vi "NetScanner.vi"() -> ()   [LabVIEW 2026]
uses:
  <vilib>/Utility/file.llb/Read From Spreadsheet File (string).vi
  <vilib>/Platform/browser.llb/Open URL in Default Browser (path).vi
panel:
  in  "Open save folder":bool
  out "Load feedback":string
  in  "Load past data:":path
  out "Dummy \nsave:":bool
  in  "selectgraph2":u16(ring)=1 caption="Plot:" items=["p/p0", "Mach"]
  in  "Mach_Chan_Select":i16=1 caption="Calculate isentropic \nMach number\nfor channel:" min=1 max=15 step=1
  out "Chan_Mach":dbl caption="Isentropic Mach number:" format="%#_3g"
  out "Saved file:":string="p_1198.csv"
  out "Folder \nchange:":bool
  in  "Ones":T1={"Ch1"=TRUE, "Ch2"=TRUE, "Ch3"=TRUE, "Ch4"=TRUE, "Ch5"=TRUE, "Ch6"=TRUE, "Ch7"=TRUE, "Ch8"=TRUE, "Ch9"=TRUE, "Ch10"=TRUE, "Ch11"=TRUE, "Ch12"=TRUE, "Ch13"=TRUE, "Ch14"=TRUE, "Ch15"=TRUE, "Ch16"=TRUE} caption="Select Channel(s)"
  in  "Zeros":T1={"Ch1"=FALSE, "Ch2"=FALSE, "Ch3"=FALSE, "Ch4"=FALSE, "Ch5"=FALSE, "Ch6"=FALSE, "Ch7"=FALSE, "Ch8"=FALSE, "Ch9"=FALSE, "Ch10"=FALSE, "Ch11"=FALSE, "Ch12"=FALSE, "Ch13"=FALSE, "Ch14"=FALSE, "Ch15"=FALSE, "Ch16"=TRUE} caption="Select Channel(s)"
  in  "Toggle 1-15":bool=TRUE
  in  "unlock":bool
  in  "Runstop":bool
  out "File prefix:":string="p"
  out "Saved":bool
  in  "Folder path:":path=path "C:/Tim/March 2026/Cont pr"
  out "run time":timestamp=timestamp(3553599339.145414 s since 1904-01-01)
  in  "TCPref":refnum<k5>
  in  "Save":bool
  in  "channelselect":T1={"Ch1"=TRUE, "Ch2"=TRUE, "Ch3"=TRUE, "Ch4"=FALSE, "Ch5"=FALSE, "Ch6"=FALSE, "Ch7"=FALSE, "Ch8"=FALSE, "Ch9"=FALSE, "Ch10"=FALSE, "Ch11"=FALSE, "Ch12"=FALSE, "Ch13"=FALSE, "Ch14"=FALSE, "Ch15"=FALSE, "Ch16"=TRUE} caption="Select Channels:"
  out "datumtime":dbl=40.092
  out "datumpressure":dbl[](array[numeric])=[-0.0017857551574707031, 0.012584686279296875, -0.003287792205810547, -0.002514362335205078, 0.0002722740173339844, 9.584426879882812e-05, 0.0011773109436035156, -0.0024390220642089844, -0.0013475418090820312, 0.00286102294921875, 0.0024023056030273438, 0.0003457069396972656, -7.152557373046875e-06, -0.00193023681640625, 0.0019822120666503906, -0.00290679931640625]
  out "graphratio":cluster{"Y":dbl[], "Y":dbl[]}[](graph)
  out "graphpressure":cluster{"Y":dbl[], "Y":dbl[]}[](graph) caption="Pressure Traces"
  in  "unitselect":u16(ring)=3 caption="View Pressures as:" items=["Absolute [kPa]", "Absolute [psi]", "Gauge [kPa]", "Gauge [psi]"]
  out "datatimes":dbl[](array[numeric])=[0.063, 0.063, 0.063, 0.063, 0.064, 0.064, 0.072, 0.082, 0.092, 0.102, 0.112, 0.122, 0.132, 0.142, 0.152, 0.162, 0.172, 0.182, 0.192, 0.202, 0.212, 0.222, 0.232, 0.242, 0.252, 0.262, 0.272, 0.282, 0.292, 0.302, 0.313, 0.322, 0.333, 0.343, 0.353, 0.363, 0.373, 0.383, 0.393, 0.403, 0.413, 0.423, 0.433, 0.443, 0.453, 0.463, 0.473, 0.483, 0.493, 0.503, 0.513, 0.523, 0.533, 0.543, 0.553, 0.563, 0.573, 0.583, 0.593, 0.603, 0.613, 0.623, 0.633, 0.643, 0.653, 0.663, 0.673, 0.683, 0.693, 0.703, 0.713, 0.723, 0.734, 0.743, 0.754, 0.764, 0.774, 0.784, 0.794, 0.804, 0.814, 0.824, 0.834, 0.844, 0.854, 0.864, 0.874, 0.884, 0.894, 0.904, 0.914, 0.924, 0.934, 0.944, 0.954, 0.964, 0.974, 0.984, 0.994, 1.004, 1.014, 1.024, 1.034, 1.044, 1.054, 1.064, 1.074, 1.084, 1.094, 1.104, 1.114, 1.125, 1.134, 1.144, 1.154, 1.164, 1.194, 1.194, 1.195, 1.205, 1.215, 1.225, 1.235, 1.245, 1.255, 1.265, 1.275, 1.285, 1.295, 1.305, 1.315, 1.325, 1.335, 1.345, 1.355, 1.365, 1.375, 1.385, 1.395, 1.405, 1.415, 1.425, 1.435, 1.445, 1.455, 1.465, 1.476, 1.485, 1.495, 1.505, 1.516, 1.525, 1.535, 1.545, 1.556, 1.566, 1.576, 1.586, 1.596, 1.606, 1.616, 1.626, 1.636, 1.646, 1.656, 1.666, 1.676, 1.686, 1.696, 1.706, 1.716, 1.726, 1.736, 1.746, 1.756, 1.766, 1.776, 1.787, 1.797, 1.807, 1.817, 1.827, 1.837, 1.847, 1.857, 1.867, 1.877, 1.887, 1.897, 1.907, 1.917, 1.927, 1.937, 1.948, 1.958, 1.967, 1.978, 1.987, 1.998, 2.008, 2.018, 2.028, 2.038, 2.048, 2.058, 2.068, 2.078, 2.088, 2.098, 2.108, 2.118, 2.128, 2.138, 2.148, 2.158, 2.168, 2.178, 2.188, 2.198, 2.208, 2.218, 2.228, 2.238, 2.248, 2.258, 2.268, 2.278, 2.288, 2.298, 2.308, 2.318, 2.328, 2.338, 2.348, 2.359, 2.368, 2.379, 2.389, 2.398, 2.409, 2.419, 2.429, 2.439, 2.449, 2.459, 2.469, 2.479, 2.489, 2.499, 2.509, 2.519, 2.529, 2.539, 2.549, 2.559, 2.569, 2.579, 2.589, 2.599, 2.609, 2.619, 2.629, 2.639, 2.649, 2.659, 2.669, 2.679, 2.689, 2.699, 2.709, 2.719, 2.729, 2.739, 2.749, 2.759, 2.769, 2.78, 2.789, 2.8, 2.809, 2.82, 2.83, 2.84, 2.85, 2.86, 2.87, 2.88, 2.89, 2.9, 2.91, 2.92, 2.93, 2.94, 2.95, 2.96, 2.97, 2.98, 2.99, 3.0, 3.01, 3.02, 3.03, 3.04, 3.05, 3.06, 3.07, 3.08, 3.09, 3.1, 3.11, 3.12, 3.13, 3.14, 3.15, 3.16, 3.17, 3.181, 3.191, 3.2, 3.21, 3.22, 3.231, 3.241, 3.251, 3.261, 3.271, 3.281, 3.291, 3.301, 3.311, 3.321, 3.331, 3.341, 3.351, 3.361, 3.371, 3.381, 3.391, 3.401, 3.411, 3.421, 3.431, 3.441, 3.451, 3.461, 3.471, 3.481, 3.491, 3.501, 3.511, 3.521, 3.531, 3.541, 3.551, 3.561, 3.571, 3.582, 3.591, 3.601, 3.611, 3.621, 3.632, 3.642, 3.652, 3.662, 3.672, 3.682, 3.692, 3.702, 3.712, 3.722, 3.732, 3.742, 3.752, 3.762, 3.772, 3.782, 3.792, 3.802, 3.812, 3.822, 3.832, 3.842, 3.852, 3.862, 3.872, 3.882, 3.892, 3.902, 3.912, 3.922, 3.932, 3.942, 3.952, 3.962, 3.972, 3.982, 3.992, 4.003, 4.012, 4.022, 4.033, 4.043, 4.053, 4.063, 4.073, 4.083, 4.093, 4.103, 4.113, 4.123, 4.133, 4.143, 4.153, 4.163, 4.173, 4.183, 4.193, 4.203, 4.213, 4.223, 4.233, 4.243, 4.253, 4.263, 4.273, 4.283, 4.293, 4.303, 4.313, 4.323, 4.333, 4.343, 4.353, 4.363, 4.373, 4.383, 4.393, 4.403, 4.414, 4.423, 4.434, 4.443, 4.453, 4.464, 4.474, 4.484, 4.494, 4.504, 4.514, 4.524, 4.534, 4.544, 4.554, 4.564, 4.574, 4.584, 4.594, 4.604, 4.614, 4.624, 4.634, 4.644, 4.654, 4.664, 4.674, 4.684, 4.694, 4.704, 4.714, 4.724, 4.734, 4.744, 4.754, 4.764, 4.774, 4.785, 4.794, 4.804, 4.814, 4.824, 4.834, 4.844, 4.854, 4.864, 4.874, 4.885, 4.895, 4.905, 4.915, 4.925, 4.935, 4.945, 4.955, 4.965, 4.975, 4.985, 4.995, 5.005, 5.015, 5.025, 5.035, 5.045, 5.055, 5.065, 5.075, 5.085, 5.095, 5.105, 5.115, 5.125, 5.135, 5.145, 5.155, 5.165, 5.175, 5.185, 5.195, 5.205, 5.215, 5.225, 5.235, 5.245, 5.256, 5.265, 5.275, 5.286, 5.295, 5.306, 5.316, 5.326, 5.336, 5.346, 5.356, 5.366, 5.376, 5.386, 5.396, 5.406, 5.416, 5.426, 5.436, 5.446, 5.456, 5.466, 5.476, 5.486, 5.496, 5.506, 5.516, 5.526, 5.536, 5.546, 5.556, 5.566, 5.576, 5.586, 5.596, 5.606, 5.616, 5.626, 5.636, 5.646, 5.656, 5.666, 5.676, 5.687, 5.696, 5.707, 5.717, 5.727, 5.737, 5.747, 5.757, 5.767, 5.777, 5.787, 5.797, 5.807, 5.817, 5.827, 5.837, 5.847, 5.857, 5.867, 5.877, 5.887, 5.897, 5.907, 5.917, 5.927, 5.937, 5.947, 5.957, 5.967, 5.977, 5.987, 5.997, 6.007, 6.017, 6.027, 6.037, 6.047, 6.057, 6.068, 6.077, 6.088, 6.097, 6.108, 6.117, 6.128, 6.138, 6.148, 6.158, 6.168, 6.178, 6.188, 6.198, 6.208, 6.218, 6.228, 6.238, 6.248, 6.258, 6.268, 6.278, 6.288, 6.298, 6.308, 6.318, 6.328, 6.338, 6.348, 6.358, 6.368, 6.378, 6.388, 6.398, 6.408, 6.418, 6.428, 6.438, 6.448, 6.458, 6.468, 6.478, 6.489, 6.498, 6.508, 6.518, 6.529, 6.538, 6.549, 6.559, 6.569, 6.579, 6.589, 6.599, 6.609, 6.619, 6.629, 6.639, 6.649, 6.659, 6.669, 6.679, 6.689, 6.699, 6.709, 6.719, 6.729, 6.739, 6.749, 6.759, 6.769, 6.779, 6.789, 6.799, 6.809, 6.819, 6.829, 6.839, 6.849, 6.859, 6.869, 6.879, 6.89, 6.899, 6.909, 6.919, 6.93, 6.939, 6.95, 6.96, 6.97, 6.98, 6.99, 7.0, 7.01, 7.02, 7.03, 7.04, 7.05, 7.06, 7.07, 7.08, 7.09, 7.1, 7.11, 7.12, 7.13, 7.14, 7.15, 7.16, 7.17, 7.18, 7.19, 7.2, 7.21, 7.22, 7.23, 7.24, 7.25, 7.26, 7.27, 7.28, 7.29, 7.3, 7.31, 7.32, 7.331, 7.341, 7.351, 7.36, 7.37, 7.381, 7.391, 7.401, 7.411, 7.421, 7.431, 7.441, 7.451, 7.461, 7.471, 7.481, 7.491, 7.501, 7.511, 7.521, 7.531, 7.541, 7.551, 7.561, 7.571, 7.581, 7.591, 7.601, 7.611, 7.621, 7.631, 7.641, 7.651, 7.661, 7.671, 7.681, 7.691, 7.701, 7.711, 7.721, 7.731, 7.741, 7.751, 7.761, 7.772, 7.782, 7.792, 7.802, 7.812, 7.822, 7.832, 7.842, 7.852, 7.862, 7.872, 7.882, 7.892, 7.902, 7.912, 7.922, 7.932, 7.942, 7.952, 7.962, 7.972, 7.982, 7.992, 8.002, 8.012, 8.022, 8.032, 8.042, 8.052, 8.062, 8.072, 8.082, 8.092, 8.102, 8.112, 8.122, 8.132, 8.142, 8.152, 8.162, 8.173, 8.183, 8.193, 8.203, 8.213, 8.223, 8.233, 8.243, 8.253, 8.263, 8.273, 8.283, 8.293, 8.303, 8.313, 8.323, 8.333, 8.343, 8.353, 8.363, 8.373, 8.383, 8.393, 8.403, 8.413, 8.423, 8.433, 8.443, 8.453, 8.463, 8.473, 8.483, 8.493, 8.503, 8.513, 8.523, 8.533, 8.543, 8.553, 8.563, 8.573, 8.583, 8.594, 8.604, 8.614, 8.624, 8.634, 8.644, 8.654, 8.664, 8.674, 8.684, 8.694, 8.704, 8.714, 8.724, 8.734, 8.744, 8.754, 8.764, 8.774, 8.784, 8.794, 8.804, 8.814, 8.824, 8.834, 8.844, 8.854, 8.864, 8.874, 8.884, 8.894, 8.904, 8.914, 8.924, 8.934, 8.944, 8.954, 8.964, 8.974, 8.984, 8.995, 9.005, 9.015, 9.025, 9.035, 9.045, 9.055, 9.065, 9.075, 9.085, 9.095, 9.105, 9.115, 9.125, 9.135, 9.145, 9.155, 9.165, 9.175, 9.185, 9.195, 9.205, 9.215, 9.225, 9.235, 9.245, 9.255, 9.265, 9.275, 9.285, 9.295, 9.305, 9.315, 9.325, 9.335, 9.345, 9.355, 9.365, 9.375, 9.385, 9.396, 9.405, 9.416, 9.426, 9.436, 9.446, 9.456, 9.466, 9.476, 9.486, 9.496, 9.506, 9.516, 9.526, 9.536, 9.546, 9.556, 9.566, 9.576, 9.586, 9.596, 9.606, 9.616, 9.626, 9.636, 9.646, 9.656, 9.666, 9.676, 9.686, 9.696, 9.706, 9.716, 9.726, 9.736, 9.746, 9.756, 9.766, 9.776, 9.786, 9.797, 9.807, 9.816, 9.827, 9.837, 9.847, 9.857, 9.867, 9.877, 9.887, 9.897, 9.907, 9.917, 9.927, 9.937, 9.947, 9.957, 9.967, 9.977, 9.987, 9.997, 10.007, 10.017, 10.027, 10.037, 10.047, 10.057, 10.067, 10.077, 10.087, 10.097, 10.107, 10.117, 10.127, 10.137, 10.147, 10.157, 10.167, 10.177, 10.187, 10.198, 10.207, 10.217, 10.227, 10.237, 10.248, 10.258, 10.268, 10.278, 10.288, 10.298, 10.308, 10.318, 10.328, 10.338, 10.348, 10.358, 10.368, 10.378, 10.388, 10.398, 10.408, 10.418, 10.428, 10.438, 10.448, 10.458, 10.468, 10.478, 10.488, 10.498, 10.508, 10.518, 10.528, 10.538, 10.548, 10.558, 10.568, 10.578, 10.588, 10.599, 10.608, 10.618, 10.628, 10.638, 10.649, 10.659, 10.669, 10.679, 10.689, 10.699, 10.709, 10.719, 10.729, 10.739, 10.749, 10.759, 10.769, 10.779, 10.789, 10.799, 10.809, 10.819, 10.829, 10.839, 10.849, 10.859, 10.869, 10.879, 10.889, 10.899, 10.909, 10.919, 10.929, 10.939, 10.949, 10.959, 10.969, 10.979, 10.989, 11.0, 11.009, 11.019, 11.029, 11.039, 11.05, 11.06, 11.07, 11.08, 11.09, 11.1, 11.11, 11.12, 11.13, 11.14, 11.15, 11.16, 11.17, 11.18, 11.19, 11.2, 11.21, 11.22, 11.23, 11.24, 11.25, 11.26, 11.27, 11.28, 11.29, 11.3, 11.31, 11.32, 11.33, 11.34, 11.35, 11.36, 11.37, 11.38, 11.39, 11.4, 11.41, 11.42, 11.43, 11.44, 11.45, 11.46, 11.47, 11.481, 11.491, 11.501, 11.511, 11.521, 11.531, 11.541, 11.551, 11.561, 11.571, 11.581, 11.591, 11.601, 11.611, 11.621, 11.631, 11.641, 11.651, 11.661, 11.671, 11.681, 11.691, 11.701, 11.711, 11.721, 11.731, 11.741, 11.751, 11.761, 11.771, 11.781, 11.791, 11.801, 11.811, 11.821, 11.831, 11.841, 11.851, 11.861, 11.871, 11.882, 11.892, 11.902, 11.912, 11.922, 11.932, 11.942, 11.952, 11.962, 11.972, 11.982, 11.992, 12.002, 12.012, 12.022, 12.032, 12.042, 12.052, 12.062, 12.072, 12.082, 12.092, 12.102, 12.112, 12.122, 12.132, 12.142, 12.152, 12.162, 12.172, 12.182, 12.192, 12.202, 12.212, 12.222, 12.232, 12.243, 12.252, 12.262, 12.272, 12.282, 12.292, 12.303, 12.313, 12.323, 12.333, 12.343, 12.353, 12.363, 12.373, 12.383, 12.393, 12.403, 12.413, 12.423, 12.433, 12.443, 12.453, 12.463, 12.473, 12.483, 12.493, 12.503, 12.513, 12.523, 12.533, 12.543, 12.553, 12.563, 12.573, 12.583, 12.593, 12.603, 12.613, 12.623, 12.633, 12.643, 12.653, 12.663, 12.673, 12.684, 12.694, 12.704, 12.714, 12.724, 12.734, 12.744, 12.754, 12.764, 12.774, 12.784, 12.794, 12.804, 12.814, 12.824, 12.834, 12.844, 12.854, 12.864, 12.874, 12.884, 12.894, 12.904, 12.914, 12.924, 12.934, 12.944, 12.954, 12.964, 12.974, 12.984, 12.994, 13.004, 13.014, 13.024, 13.034, 13.044, 13.054, 13.064, 13.074, 13.084, 13.094, 13.104, 13.115, 13.125, 13.135, 13.145, 13.155, 13.165, 13.175, 13.185, 13.195, 13.205, 13.215, 13.225, 13.235, 13.245, 13.255, 13.265, 13.275, 13.285, 13.295, 13.305, 13.315, 13.325, 13.335, 13.345, 13.355, 13.365, 13.375, 13.385, 13.395, 13.405, 13.415, 13.425, 13.435, 13.445, 13.455, 13.465, 13.475, 13.485, 13.495, 13.506, 13.515, 13.525, 13.536, 13.546, 13.556, 13.566, 13.576, 13.586, 13.596, 13.606, 13.616, 13.626, 13.636, 13.646, 13.656, 13.666, 13.676, 13.686, 13.696, 13.706, 13.716, 13.726, 13.736, 13.746, 13.756, 13.766, 13.776, 13.786, 13.796, 13.806, 13.816, 13.826, 13.836, 13.846, 13.856, 13.866, 13.876, 13.886, 13.896, 13.906, 13.916, 13.926, 13.936, 13.946, 13.956, 13.966, 13.977, 13.987, 13.997, 14.007, 14.017, 14.027, 14.037, 14.047, 14.057, 14.067, 14.077, 14.087, 14.097, 14.107, 14.117, 14.127, 14.137, 14.147, 14.157, 14.167, 14.177, 14.187, 14.197, 14.207, 14.217, 14.227, 14.237, 14.247, 14.257, 14.267, 14.277, 14.287, 14.297, 14.307, 14.317, 14.327, 14.338, 14.348, 14.357, 14.368, 14.378, 14.388, 14.398, 14.408, 14.418, 14.428, 14.438, 14.448, 14.458, 14.468, 14.478, 14.488, 14.498, 14.508, 14.518, 14.528, 14.538, 14.548, 14.558, 14.568, 14.578, 14.588, 14.598, 14.608, 14.618, 14.628, 14.638, 14.648, 14.658, 14.668, 14.678, 14.688, 14.698, 14.708, 14.718, 14.728, 14.739, 14.749, 14.759, 14.769, 14.779, 14.789, 14.799, 14.809, 14.819, 14.829, 14.839, 14.849, 14.859, 14.869, 14.879, 14.889, 14.899, 14.909, 14.919, 14.929, 14.939, 14.949, 14.959, 14.969, 14.979, 14.989, 14.999, 15.009, 15.019, 15.029, 15.039, 15.049, 15.059, 15.069, 15.079, 15.089, 15.099, 15.109, 15.12, 15.13, 15.14, 15.15, 15.16, 15.17, 15.18, 15.19, 15.2, 15.21, 15.22, 15.23, 15.24, 15.25, 15.26, 15.27, 15.28, 15.29, 15.3, 15.31, 15.32, 15.33, 15.34, 15.35, 15.36, 15.37, 15.38, 15.39, 15.4, 15.446, 15.446, 15.446, 15.446, 15.45, 15.46, 15.47, 15.48, 15.49, 15.5, 15.51, 15.52, 15.53, 15.54, 15.55, 15.56, 15.571, 15.581, 15.591, 15.601, 15.611, 15.621, 15.631, 15.641, 15.651, 15.661, 15.671, 15.681, 15.691, 15.701, 15.711, 15.721, 15.731, 15.741, 15.751, 15.761, 15.771, 15.781, 15.791, 15.801, 15.811, 15.821, 15.831, 15.841, 15.851, 15.861, 15.871, 15.881, 15.891, 15.901, 15.911, 15.922, 15.931, 15.941, 15.951, 15.962, 15.972, 15.982, 15.992, 16.002, 16.012, 16.022, 16.032, 16.042, 16.052, 16.062, 16.072, 16.082, 16.092, 16.102, 16.112, 16.122, 16.132, 16.142, 16.152, 16.162, 16.172, 16.182, 16.192, 16.202, 16.212, 16.222, 16.232, 16.242, 16.252, 16.262, 16.272, 16.282, 16.292, 16.302, 16.312, 16.322, 16.332, 16.342, 16.352, 16.362, 16.372, 16.382, 16.392, 16.402, 16.413, 16.423, 16.433, 16.443, 16.453, 16.463, 16.473, 16.483, 16.493, 16.503, 16.513, 16.523, 16.533, 16.543, 16.553, 16.563, 16.573, 16.583, 16.593, 16.603, 16.613, 16.623, 16.633, 16.643, 16.653, 16.663, 16.673, 16.683, 16.693, 16.703, 16.713, 16.723, 16.733, 16.743, 16.753, 16.763, 16.773, 16.784, 16.793, 16.804, 16.814, 16.824, 16.834, 16.844, 16.854, 16.864, 16.874, 16.884, 16.894, 16.904, 16.914, 16.924, 16.934, 16.944, 16.954, 16.964, 16.974, 16.984, 16.994, 17.004, 17.014, 17.024, 17.034, 17.044, 17.054, 17.064, 17.074, 17.084, 17.094, 17.104, 17.114, 17.124, 17.134, 17.144, 17.154, 17.164, 17.174, 17.184, 17.194, 17.205, 17.215, 17.225, 17.235, 17.245, 17.255, 17.264, 17.275, 17.285, 17.295, 17.305, 17.315, 17.325, 17.335, 17.345, 17.355, 17.365, 17.375, 17.385, 17.395, 17.405, 17.415, 17.425, 17.435, 17.445, 17.455, 17.465, 17.475, 17.485, 17.495, 17.505, 17.515, 17.525, 17.535, 17.545, 17.556, 17.565, 17.575, 17.586, 17.596, 17.605, 17.616, 17.626, 17.636, 17.646, 17.656, 17.666, 17.676, 17.686, 17.696, 17.706, 17.716, 17.726, 17.736, 17.746, 17.756, 17.766, 17.776, 17.786, 17.796, 17.806, 17.816, 17.826, 17.836, 17.846, 17.856, 17.866, 17.876, 17.886, 17.896, 17.906, 17.916, 17.926, 17.936, 17.946, 17.957, 17.966, 17.976, 17.986, 17.996, 18.007, 18.017, 18.027, 18.037, 18.047, 18.057, 18.067, 18.077, 18.087, 18.097, 18.107, 18.117, 18.127, 18.137, 18.147, 18.157, 18.167, 18.177, 18.187, 18.197, 18.207, 18.217, 18.227, 18.237, 18.247, 18.257, 18.267, 18.277, 18.287, 18.297, 18.307, 18.317, 18.327, 18.337, 18.347, 18.357, 18.367, 18.377, 18.387, 18.397, 18.407, 18.418, 18.427, 18.438, 18.447, 18.457, 18.467, 18.478, 18.488, 18.498, 18.508, 18.518, 18.528, 18.538, 18.548, 18.558, 18.568, 18.578, 18.588, 18.598, 18.608, 18.618, 18.628, 18.638, 18.648, 18.658, 18.668, 18.678, 18.688, 18.698, 18.708, 18.718, 18.728, 18.738, 18.748, 18.758, 18.768, 18.778, 18.788, 18.798, 18.808, 18.818, 18.828, 18.838, 18.848, 18.858, 18.868, 18.878, 18.889, 18.899, 18.909, 18.919, 18.929, 18.939, 18.949, 18.959, 18.969, 18.979, 18.989, 18.999, 19.009, 19.019, 19.029, 19.039, 19.049, 19.059, 19.069, 19.079, 19.089, 19.099, 19.109, 19.119, 19.129, 19.139, 19.149, 19.159, 19.169, 19.179, 19.189, 19.199, 19.209, 19.219, 19.23, 19.24, 19.249, 19.259, 19.27, 19.28, 19.29, 19.301, 19.31, 19.321, 19.331, 19.341, 19.351, 19.361, 19.371, 19.381, 19.391, 19.401, 19.411, 19.421, 19.431, 19.441, 19.451, 19.461, 19.471, 19.481, 19.491, 19.501, 19.511, 19.521, 19.531, 19.541, 19.551, 19.561, 19.571, 19.581, 19.591, 19.601, 19.611, 19.622, 19.631, 19.641, 19.651, 19.661, 19.671, 19.681, 19.691, 19.701, 19.711, 19.722, 19.731, 19.741, 19.751, 19.762, 19.772, 19.782, 19.792, 19.802, 19.812, 19.822, 19.832, 19.842, 19.852, 19.862, 19.872, 19.882, 19.892, 19.902, 19.912, 19.922, 19.932, 19.942, 19.952, 19.962, 19.972, 19.982, 19.992, 20.002, 20.012, 20.022, 20.032, 20.042, 20.052, 20.062, 20.072, 20.082, 20.092, 20.102, 20.112, 20.122, 20.132, 20.143, 20.153, 20.163, 20.173, 20.183, 20.193, 20.203, 20.213, 20.223, 20.233, 20.243, 20.253, 20.263, 20.273, 20.283, 20.293, 20.303, 20.313, 20.323, 20.333, 20.343, 20.353, 20.363, 20.373, 20.383, 20.393, 20.403, 20.413, 20.423, 20.433, 20.443, 20.453, 20.463, 20.473, 20.483, 20.493, 20.503, 20.513, 20.523, 20.533, 20.544, 20.554, 20.564, 20.574, 20.584, 20.594, 20.604, 20.614, 20.624, 20.634, 20.644, 20.654, 20.664, 20.674, 20.684, 20.694, 20.704, 20.714, 20.724, 20.734, 20.744, 20.754, 20.764, 20.774, 20.784, 20.794, 20.804, 20.814, 20.824, 20.834, 20.844, 20.854, 20.864, 20.874, 20.884, 20.894, 20.904, 20.914, 20.925, 20.934, 20.944, 20.954, 20.964, 20.975, 20.985, 20.995, 21.005, 21.015, 21.025, 21.035, 21.045, 21.055, 21.065, 21.075, 21.085, 21.095, 21.105, 21.115, 21.125, 21.135, 21.145, 21.155, 21.165, 21.175, 21.185, 21.195, 21.205, 21.215, 21.225, 21.235, 21.245, 21.255, 21.265, 21.275, 21.285, 21.295, 21.305, 21.315, 21.325, 21.335, 21.345, 21.355, 21.366, 21.376, 21.386, 21.396, 21.406, 21.416, 21.426, 21.436, 21.446, 21.456, 21.466, 21.476, 21.486, 21.496, 21.506, 21.516, 21.526, 21.536, 21.546, 21.556, 21.566, 21.576, 21.586, 21.596, 21.606, 21.616, 21.626, 21.636, 21.646, 21.656, 21.666, 21.676, 21.686, 21.696, 21.706, 21.716, 21.726, 21.736, 21.746, 21.756, 21.766, 21.776, 21.786, 21.796, 21.806, 21.817, 21.826, 21.837, 21.847, 21.857, 21.867, 21.877, 21.887, 21.897, 21.907, 21.917, 21.927, 21.937, 21.947, 21.957, 21.967, 21.977, 21.987, 21.997, 22.007, 22.017, 22.027, 22.037, 22.047, 22.057, 22.067, 22.077, 22.087, 22.097, 22.107, 22.118, 22.127, 22.137, 22.147, 22.157, 22.167, 22.177, 22.188, 22.198, 22.208, 22.218, 22.228, 22.238, 22.248, 22.258, 22.268, 22.278, 22.288, 22.298, 22.308, 22.318, 22.328, 22.338, 22.348, 22.358, 22.368, 22.378, 22.388, 22.398, 22.408, 22.418, 22.428, 22.438, 22.448, 22.458, 22.468, 22.478, 22.488, 22.498, 22.508, 22.518, 22.528, 22.538, 22.548, 22.558, 22.568, 22.579, 22.589, 22.599, 22.609, 22.619, 22.629, 22.639, 22.649, 22.659, 22.669, 22.679, 22.689, 22.699, 22.709, 22.719, 22.729, 22.739, 22.749, 22.759, 22.769, 22.779, 22.789, 22.799, 22.809, 22.819, 22.829, 22.839, 22.849, 22.859, 22.869, 22.879, 22.889, 22.899, 22.909, 22.919, 22.929, 22.939, 22.949, 22.959, 22.969, 22.979, 22.989, 22.999, 23.009, 23.019, 23.03, 23.039, 23.049, 23.059, 23.07, 23.08, 23.09, 23.1, 23.11, 23.12, 23.13, 23.14, 23.15, 23.16, 23.17, 23.18, 23.19, 23.2, 23.21, 23.22, 23.23, 23.24, 23.25, 23.26, 23.27, 23.28, 23.29, 23.3, 23.31, 23.32, 23.33, 23.34, 23.35, 23.36, 23.37, 23.38, 23.39, 23.4, 23.41, 23.42, 23.43, 23.441, 23.45, 23.461, 23.471, 23.481, 23.491, 23.501, 23.511, 23.521, 23.531, 23.541, 23.551, 23.561, 23.571, 23.581, 23.591, 23.601, 23.611, 23.621, 23.631, 23.641, 23.651, 23.661, 23.671, 23.681, 23.691, 23.701, 23.711, 23.721, 23.731, 23.741, 23.751, 23.761, 23.771, 23.781, 23.791, 23.801, 23.811, 23.821, 23.831, 23.841, 23.851, 23.861, 23.871, 23.882, 23.892, 23.902, 23.912, 23.922, 23.932, 23.942, 23.952, 23.962, 23.972, 23.982, 23.992, 24.002, 24.012, 24.022, 24.032, 24.042, 24.052, 24.062, 24.072, 24.082, 24.092, 24.102, 24.112, 24.122, 24.132, 24.142, 24.152, 24.162, 24.172, 24.182, 24.192, 24.202, 24.212, 24.222, 24.232, 24.242, 24.252, 24.262, 24.272, 24.282, 24.292, 24.303, 24.313, 24.323, 24.333, 24.343, 24.353, 24.363, 24.373, 24.383, 24.393, 24.403, 24.413, 24.423, 24.433, 24.443, 24.453, 24.463, 24.473, 24.483, 24.493, 24.503, 24.513, 24.523, 24.533, 24.543, 24.553, 24.563, 24.573, 24.583, 24.593, 24.603, 24.613, 24.623, 24.633, 24.643, 24.654, 24.663, 24.674, 24.684, 24.693, 24.703, 24.714, 24.724, 24.734, 24.744, 24.754, 24.764, 24.774, 24.784, 24.794, 24.804, 24.814, 24.824, 24.834, 24.844, 24.854, 24.864, 24.874, 24.884, 24.894, 24.904, 24.914, 24.924, 24.934, 24.944, 24.954, 24.964, 24.974, 24.984, 24.994, 25.004, 25.014, 25.024, 25.034, 25.044, 25.054, 25.064, 25.075, 25.084, 25.094, 25.105, 25.115, 25.125, 25.135, 25.145, 25.155, 25.165, 25.175, 25.185, 25.195, 25.205, 25.215, 25.225, 25.235, 25.245, 25.255, 25.265, 25.275, 25.285, 25.295, 25.305, 25.315, 25.325, 25.335, 25.345, 25.355, 25.365, 25.375, 25.385, 25.395, 25.405, 25.415, 25.425, 25.435, 25.445, 25.456, 25.466, 25.476, 25.486, 25.496, 25.506, 25.516, 25.526, 25.536, 25.546, 25.556, 25.566, 25.576, 25.586, 25.596, 25.606, 25.616, 25.626, 25.636, 25.646, 25.656, 25.666, 25.676, 25.686, 25.696, 25.706, 25.716, 25.726, 25.736, 25.746, 25.756, 25.766, 25.776, 25.786, 25.796, 25.806, 25.816, 25.826, 25.836, 25.846, 25.856, 25.866, 25.876, 25.886, 25.896, 25.907, 25.916, 25.927, 25.937, 25.947, 25.957, 25.967, 25.977, 25.987, 25.997, 26.007, 26.017, 26.027, 26.037, 26.047, 26.057, 26.067, 26.077, 26.087, 26.097, 26.107, 26.117, 26.127, 26.137, 26.147, 26.157, 26.167, 26.177, 26.187, 26.197, 26.207, 26.217, 26.227, 26.237, 26.247, 26.257, 26.267, 26.277, 26.287, 26.297, 26.307, 26.317, 26.328, 26.338, 26.348, 26.358, 26.367, 26.378, 26.388, 26.398, 26.408, 26.418, 26.428, 26.438, 26.448, 26.458, 26.468, 26.478, 26.488, 26.498, 26.508, 26.518, 26.528, 26.538, 26.548, 26.558, 26.568, 26.578, 26.588, 26.598, 26.608, 26.618, 26.628, 26.638, 26.648, 26.658, 26.668, 26.678, 26.688, 26.698, 26.708, 26.718, 26.728, 26.738, 26.748, 26.758, 26.769, 26.779, 26.789, 26.799, 26.809, 26.819, 26.829, 26.839, 26.849, 26.859, 26.869, 26.879, 26.889, 26.899, 26.909, 26.919, 26.929, 26.939, 26.949, 26.959, 26.969, 26.979, 26.989, 26.999, 27.009, 27.019, 27.029, 27.039, 27.049, 27.059, 27.069, 27.079, 27.089, 27.099, 27.109, 27.119, 27.129, 27.139, 27.149, 27.159, 27.169, 27.18, 27.19, 27.2, 27.209, 27.22, 27.23, 27.24, 27.25, 27.26, 27.27, 27.28, 27.29, 27.3, 27.31, 27.321, 27.33, 27.34, 27.35, 27.36, 27.37, 27.38, 27.39, 27.4, 27.41, 27.42, 27.43, 27.44, 27.45, 27.46, 27.47, 27.48, 27.49, 27.5, 27.51, 27.52, 27.53, 27.54, 27.55, 27.56, 27.57, 27.58, 27.591, 27.601, 27.611, 27.62, 27.631, 27.641, 27.651, 27.661, 27.671, 27.681, 27.691, 27.701, 27.713, 27.721, 27.731, 27.741, 27.751, 27.761, 27.771, 27.781, 27.791, 27.801, 27.811, 27.821, 27.831, 27.841, 27.851, 27.861, 27.871, 27.881, 27.891, 27.901, 27.911, 27.921, 27.931, 27.941, 27.951, 27.961, 27.971, 27.981, 27.991, 28.002, 28.011, 28.021, 28.031, 28.042, 28.052, 28.062, 28.072, 28.082, 28.092, 28.102, 28.112, 28.122, 28.132, 28.142, 28.152, 28.162, 28.172, 28.182, 28.192, 28.202, 28.212, 28.222, 28.232, 28.242, 28.252, 28.262, 28.272, 28.282, 28.292, 28.302, 28.312, 28.322, 28.332, 28.342, 28.352, 28.362, 28.372, 28.382, 28.392, 28.402, 28.412, 28.423, 28.432, 28.443, 28.452, 28.463, 28.473, 28.483, 28.493, 28.503, 28.513, 28.523, 28.533, 28.543, 28.553, 28.563, 28.573, 28.583, 28.593, 28.603, 28.613, 28.623, 28.633, 28.643, 28.653, 28.663, 28.673, 28.683, 28.693, 28.703, 28.713, 28.723, 28.733, 28.743, 28.753, 28.763, 28.774, 28.783, 28.793, 28.803, 28.814, 28.824, 28.833, 28.843, 28.854, 28.864, 28.874, 28.884, 28.894, 28.904, 28.914, 28.924, 28.934, 28.944, 28.954, 28.964, 28.974, 28.984, 28.994, 29.004, 29.014, 29.024, 29.034, 29.044, 29.054, 29.064, 29.074, 29.084, 29.094, 29.104, 29.114, 29.124, 29.134, 29.144, 29.154, 29.165, 29.174, 29.185, 29.195, 29.205, 29.215, 29.225, 29.235, 29.245, 29.255, 29.265, 29.275, 29.285, 29.295, 29.305, 29.315, 29.325, 29.335, 29.345, 29.355, 29.365, 29.375, 29.385, 29.395, 29.405, 29.415, 29.425, 29.435, 29.445, 29.455, 29.465, 29.475, 29.485, 29.495, 29.505, 29.515, 29.525, 29.535, 29.545, 29.556, 29.565, 29.575, 29.586, 29.596, 29.606, 29.616, 29.626, 29.636, 29.646, 29.656, 29.666, 29.676, 29.686, 29.696, 29.706, 29.716, 29.726, 29.736, 29.746, 29.756, 29.766, 29.776, 29.786, 29.796, 29.806, 29.816, 29.826, 29.836, 29.846, 29.856, 29.866, 29.876, 29.886, 29.896, 29.906, 29.916, 29.926, 29.936, 29.946, 29.957, 29.966, 29.976, 29.986, 29.996, 30.006, 30.017, 30.027, 30.037, 30.047, 30.057, 30.067, 30.077, 30.087, 30.097, 30.107, 30.117, 30.127, 30.137, 30.147, 30.157, 30.167, 30.177, 30.187, 30.197, 30.207, 30.217, 30.227, 30.237, 30.247, 30.257, 30.267, 30.277, 30.287, 30.297, 30.308, 30.317, 30.327, 30.337, 30.347, 30.358, 30.367, 30.378, 30.388, 30.398, 30.408, 30.417, 30.428, 30.438, 30.448, 30.458, 30.468, 30.478, 30.488, 30.498, 30.508, 30.518, 30.528, 30.538, 30.548, 30.558, 30.568, 30.578, 30.588, 30.598, 30.608, 30.618, 30.628, 30.638, 30.648, 30.658, 30.668, 30.678, 30.688, 30.698, 30.708, 30.718, 30.728, 30.738, 30.748, 30.758, 30.768, 30.778, 30.788, 30.798, 30.808, 30.818, 30.829, 30.839, 30.849, 30.859, 30.869, 30.879, 30.889, 30.899, 30.909, 30.919, 30.929, 30.939, 30.949, 30.959, 30.969, 30.979, 30.989, 30.999, 31.009, 31.019, 31.029, 31.039, 31.049, 31.059, 31.069, 31.079, 31.089, 31.099, 31.109, 31.119, 31.129, 31.139, 31.149, 31.159, 31.169, 31.179, 31.189, 31.199, 31.21, 31.219, 31.23, 31.24, 31.25, 31.26, 31.269, 31.28, 31.29, 31.3, 31.31, 31.32, 31.33, 31.34, 31.35, 31.36, 31.37, 31.38, 31.39, 31.4, 31.41, 31.42, 31.43, 31.44, 31.45, 31.46, 31.47, 31.48, 31.49, 31.5, 31.51, 31.52, 31.53, 31.54, 31.55, 31.56, 31.57, 31.58, 31.59, 31.6, 31.61, 31.62, 31.63, 31.64, 31.651, 31.661, 31.671, 31.681, 31.691, 31.701, 31.711, 31.721, 31.731, 31.741, 31.751, 31.761, 31.771, 31.781, 31.791, 31.801, 31.811, 31.821, 31.831, 31.841, 31.851, 31.861, 31.871, 31.881, 31.891, 31.901, 31.911, 31.921, 31.932, 31.941, 31.951, 31.961, 31.971, 31.981, 31.991, 32.001, 32.011, 32.021, 32.031, 32.041, 32.051, 32.062, 32.072, 32.082, 32.092, 32.102, 32.112, 32.122, 32.132, 32.142, 32.152, 32.162, 32.172, 32.182, 32.192, 32.202, 32.212, 32.222, 32.232, 32.242, 32.252, 32.262, 32.272, 32.282, 32.292, 32.302, 32.312, 32.322, 32.332, 32.342, 32.352, 32.363, 32.372, 32.382, 32.392, 32.402, 32.412, 32.422, 32.432, 32.442, 32.452, 32.462, 32.472, 32.482, 32.492, 32.502, 32.512, 32.523, 32.533, 32.543, 32.553, 32.562, 32.573, 32.583, 32.593, 32.603, 32.613, 32.623, 32.633, 32.643, 32.653, 32.663, 32.673, 32.683, 32.693, 32.703, 32.713, 32.723, 32.733, 32.743, 32.753, 32.763, 32.773, 32.783, 32.793, 32.803, 32.813, 32.823, 32.833, 32.843, 32.853, 32.863, 32.873, 32.884, 32.894, 32.904, 32.914, 32.924, 32.934, 32.944, 32.954, 32.964, 32.974, 32.984, 32.994, 33.004, 33.014, 33.024, 33.034, 33.044, 33.054, 33.064, 33.074, 33.084, 33.094, 33.104, 33.114, 33.124, 33.134, 33.144, 33.154, 33.164, 33.174, 33.184, 33.194, 33.204, 33.214, 33.224, 33.234, 33.244, 33.254, 33.264, 33.274, 33.284, 33.294, 33.304, 33.315, 33.324, 33.334, 33.344, 33.355, 33.365, 33.375, 33.385, 33.395, 33.405, 33.415, 33.425, 33.435, 33.445, 33.455, 33.465, 33.475, 33.485, 33.495, 33.505, 33.515, 33.525, 33.535, 33.545, 33.555, 33.565, 33.575, 33.585, 33.595, 33.605, 33.615, 33.625, 33.635, 33.645, 33.655, 33.665, 33.675, 33.685, 33.695, 33.705, 33.715, 33.725, 33.735, 33.745, 33.756, 33.765, 33.775, 33.786, 33.796, 33.806, 33.816, 33.826, 33.836, 33.846, 33.856, 33.866, 33.876, 33.886, 33.896, 33.906, 33.916, 33.926, 33.936, 33.946, 33.956, 33.966, 33.976, 33.986, 33.996, 34.006, 34.016, 34.026, 34.036, 34.046, 34.056, 34.066, 34.076, 34.086, 34.096, 34.106, 34.116, 34.126, 34.136, 34.146, 34.156, 34.166, 34.176, 34.186, 34.197, 34.206, 34.216, 34.226, 34.237, 34.247, 34.257, 34.267, 34.277, 34.287, 34.297, 34.307, 34.317, 34.327, 34.337, 34.347, 34.357, 34.367, 34.377, 34.387, 34.397, 34.407, 34.417, 34.427, 34.437, 34.447, 34.457, 34.467, 34.477, 34.487, 34.497, 34.507, 34.517, 34.527, 34.537, 34.547, 34.557, 34.567, 34.577, 34.587, 34.597, 34.607, 34.617, 34.628, 34.638, 34.648, 34.658, 34.668, 34.678, 34.688, 34.698, 34.708, 34.718, 34.728, 34.738, 34.748, 34.758, 34.768, 34.778, 34.788, 34.798, 34.808, 34.818, 34.828, 34.838, 34.848, 34.858, 34.868, 34.878, 34.888, 34.898, 34.908, 34.918, 34.928, 34.938, 34.948, 34.958, 34.968, 34.978, 34.988, 34.998, 35.008, 35.018, 35.029, 35.039, 35.049, 35.059, 35.069, 35.079, 35.089, 35.099, 35.109, 35.119, 35.129, 35.139, 35.149, 35.159, 35.169, 35.179, 35.189, 35.199, 35.209, 35.219, 35.229, 35.239, 35.249, 35.259, 35.269, 35.279, 35.289, 35.299, 35.309, 35.319, 35.329, 35.339, 35.349, 35.359, 35.369, 35.379, 35.389, 35.399, 35.409, 35.419, 35.429, 35.44, 35.449, 35.46, 35.469, 35.48, 35.49, 35.5, 35.51, 35.52, 35.53, 35.54, 35.55, 35.56, 35.57, 35.58, 35.59, 35.6, 35.61, 35.62, 35.63, 35.64, 35.65, 35.66, 35.671, 35.68, 35.69, 35.7, 35.71, 35.72, 35.73, 35.74, 35.75, 35.761, 35.77, 35.781, 35.791, 35.801, 35.811, 35.821, 35.831, 35.841, 35.85, 35.861, 35.871, 35.881, 35.891, 35.901, 35.911, 35.921, 35.931, 35.941, 35.951, 35.961, 35.971, 35.981, 35.991, 36.001, 36.011, 36.021, 36.031, 36.041, 36.051, 36.061, 36.071, 36.081, 36.091, 36.101, 36.111, 36.121, 36.131, 36.141, 36.151, 36.161, 36.171, 36.181, 36.191, 36.201, 36.211, 36.222, 36.231, 36.241, 36.252, 36.262, 36.272, 36.282, 36.292, 36.302, 36.312, 36.322, 36.332, 36.342, 36.352, 36.362, 36.372, 36.382, 36.392, 36.402, 36.412, 36.422, 36.432, 36.442, 36.452, 36.462, 36.472, 36.482, 36.492, 36.502, 36.512, 36.522, 36.532, 36.542, 36.552, 36.562, 36.572, 36.582, 36.592, 36.602, 36.612, 36.622, 36.632, 36.642, 36.653, 36.663, 36.673, 36.682, 36.693, 36.703, 36.713, 36.723, 36.733, 36.743, 36.754, 36.764, 36.774, 36.784, 36.794, 36.804, 36.814, 36.824, 36.834, 36.844, 36.854, 36.864, 36.874, 36.884, 36.894, 36.904, 36.914, 36.924, 36.934, 36.944, 36.954, 36.964, 36.974, 36.984, 36.994, 37.004, 37.014, 37.024, 37.034, 37.044, 37.054, 37.064, 37.074, 37.084, 37.095, 37.105, 37.115, 37.125, 37.135, 37.145, 37.155, 37.165, 37.175, 37.185, 37.195, 37.205, 37.215, 37.225, 37.235, 37.245, 37.255, 37.265, 37.275, 37.285, 37.295, 37.305, 37.315, 37.325, 37.335, 37.345, 37.355, 37.365, 37.375, 37.385, 37.395, 37.405, 37.415, 37.425, 37.435, 37.446, 37.455, 37.465, 37.476, 37.486, 37.496, 37.506, 37.516, 37.526, 37.536, 37.546, 37.556, 37.566, 37.576, 37.586, 37.596, 37.606, 37.616, 37.626, 37.636, 37.646, 37.656, 37.666, 37.676, 37.686, 37.696, 37.706, 37.716, 37.726, 37.736, 37.746, 37.756, 37.766, 37.776, 37.786, 37.796, 37.806, 37.816, 37.826, 37.836, 37.846, 37.856, 37.866, 37.877, 37.886, 37.897, 37.907, 37.917, 37.927, 37.937, 37.947, 37.957, 37.967, 37.977, 37.987, 37.997, 38.007, 38.017, 38.027, 38.037, 38.047, 38.057, 38.067, 38.077, 38.087, 38.097, 38.107, 38.117, 38.127, 38.137, 38.147, 38.157, 38.167, 38.177, 38.187, 38.197, 38.207, 38.217, 38.227, 38.237, 38.247, 38.257, 38.267, 38.277, 38.287, 38.297, 38.307, 38.318, 38.328, 38.338, 38.348, 38.358, 38.368, 38.378, 38.388, 38.398, 38.408, 38.418, 38.428, 38.438, 38.448, 38.458, 38.468, 38.478, 38.488, 38.498, 38.508, 38.518, 38.528, 38.538, 38.548, 38.558, 38.568, 38.578, 38.588, 38.598, 38.608, 38.618, 38.628, 38.638, 38.648, 38.658, 38.668, 38.678, 38.688, 38.698, 38.708, 38.719, 38.729, 38.739, 38.749, 38.759, 38.769, 38.779, 38.789, 38.799, 38.809, 38.819, 38.829, 38.839, 38.849, 38.859, 38.869, 38.879, 38.889, 38.899, 38.909, 38.919, 38.929, 38.939, 38.949, 38.959, 38.969, 38.979, 38.989, 38.999, 39.009, 39.019, 39.029, 39.039, 39.049, 39.059, 39.069, 39.079, 39.089, 39.099, 39.109, 39.119, 39.129, 39.14, 39.15, 39.16, 39.17, 39.18, 39.19, 39.2, 39.21, 39.22, 39.23, 39.24, 39.25, 39.26, 39.27, 39.28, 39.29, 39.3, 39.31, 39.32, 39.33, 39.34, 39.35, 39.36, 39.37, 39.38, 39.39, 39.4, 39.41, 39.42, 39.43, 39.44, 39.45, 39.46, 39.47, 39.48, 39.49, 39.501, 39.51, 39.52, 39.53, 39.541, 39.551, 39.561, 39.571, 39.581, 39.591, 39.601, 39.611, 39.621, 39.631, 39.641, 39.651, 39.661, 39.671, 39.681, 39.691, 39.701, 39.711, 39.721, 39.731, 39.741, 39.751, 39.761, 39.771, 39.781, 39.791, 39.801, 39.811, 39.821, 39.831, 39.841, 39.851, 39.861, 39.871, 39.881, 39.891, 39.901, 39.911, 39.921, 39.931, 39.941, 39.952, 39.961, 39.972, 39.982, 39.992, 40.002, 40.012, 40.022, 40.032, 40.042, 40.052, 40.062, 40.072, 40.082, 40.092]
  out "datapressure":dbl[][](array[numeric])
  out "Missed Packets":i8
  out "Running":bool
  in  "Run":bool
  in  "atmpressure":dbl=30.17 caption="Barometric pressure" min=0.0 step=0.001
  in  "timeinterval":i32=10 caption="Sampling interval:" min=0 max=1000 step=5
  in  "timetotal":dbl=120.0 caption="Max run time:" min=1.0 step=1.0
  out "Connected":bool
  in  "EndVI":bool
  in  "Connect":bool=TRUE
  in  "Rezero":bool
  out "Samples Collected":i32=3999
  out "Rezero Values":dbl[](array[numeric]) format="%.5f"
  in  "IP Address":string="200.200.34.24"
  # "in Hg"
  # "seconds"
  # "ms"
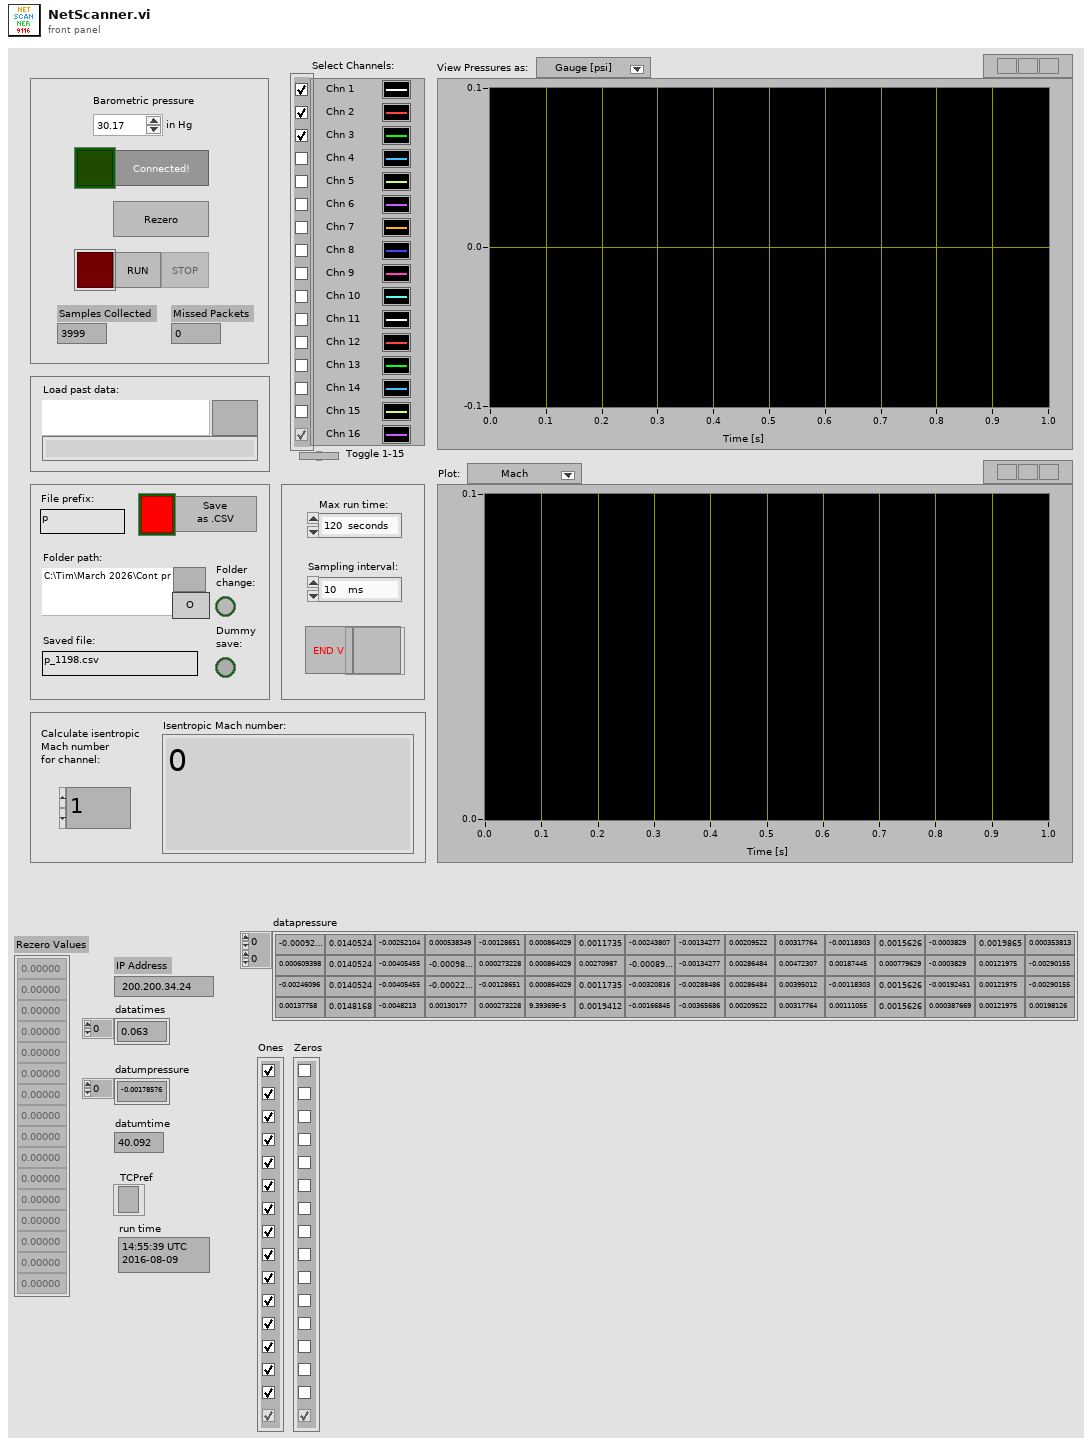
[diagram p1: front panel]
types:
  T1 = cluster{"Ch1":bool, "Ch2":bool, "Ch3":bool, "Ch4":bool, "Ch5":bool, "Ch6":bool, "Ch7":bool, "Ch8":bool, "Ch9":bool, "Ch10":bool, "Ch11":bool, "Ch12":bool, "Ch13":bool, "Ch14":bool, "Ch15":bool, "Ch16":bool}
  T2 = enum8{"Enabled", "Disabled", "Disabled and Grayed Out"}
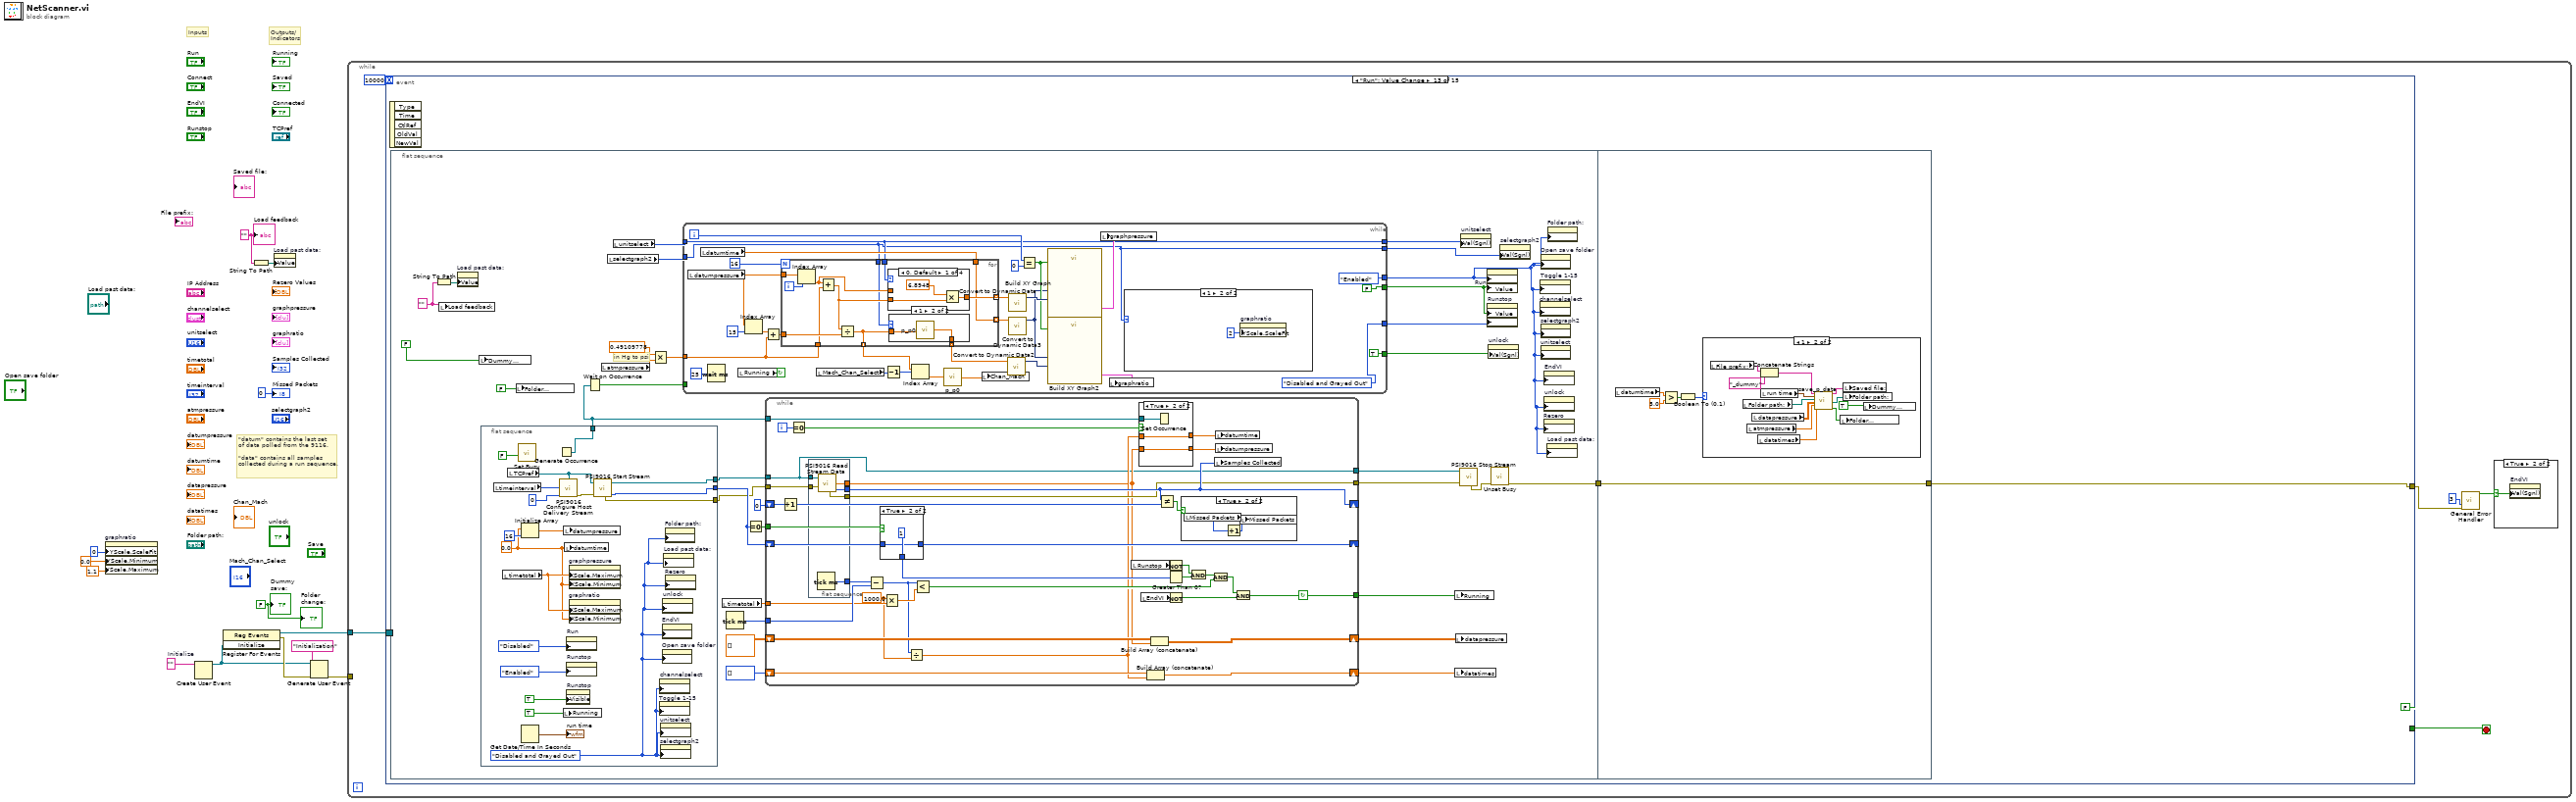
[diagram p0: block diagram]
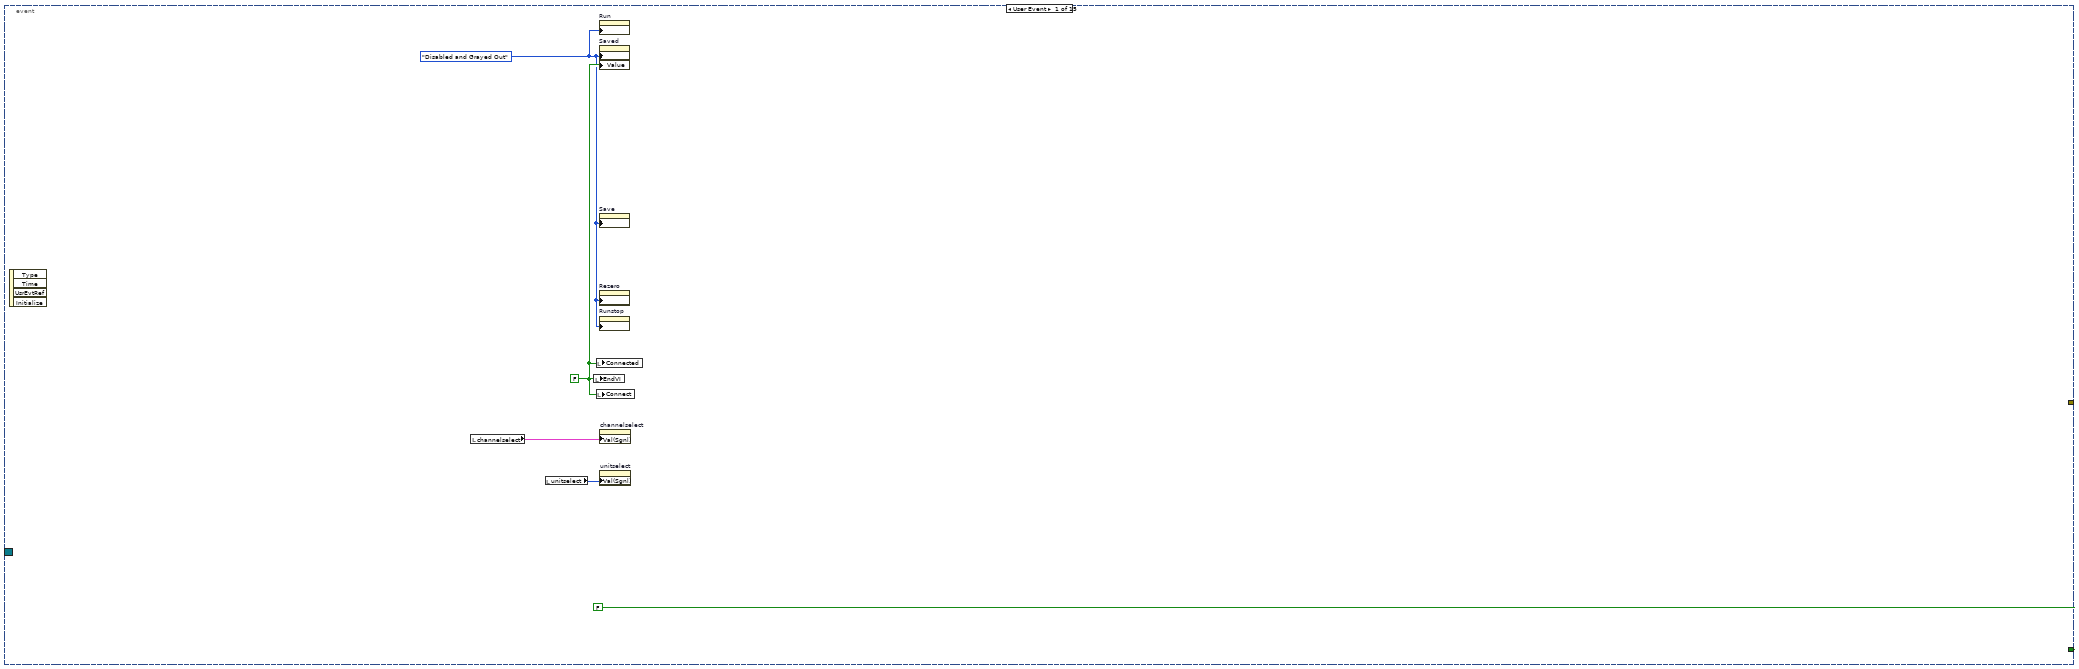
[diagram p3: hidden frame]
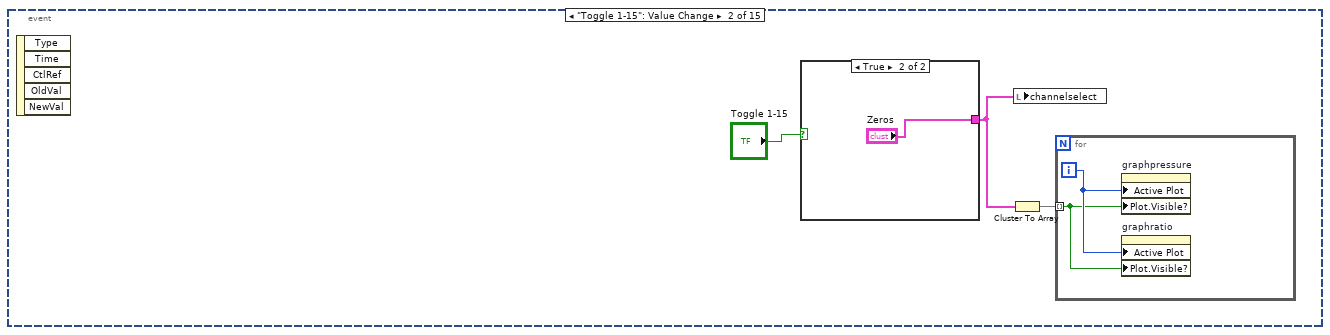
[diagram p4: hidden frame]
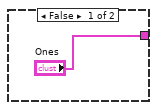
[diagram p5: hidden frame]
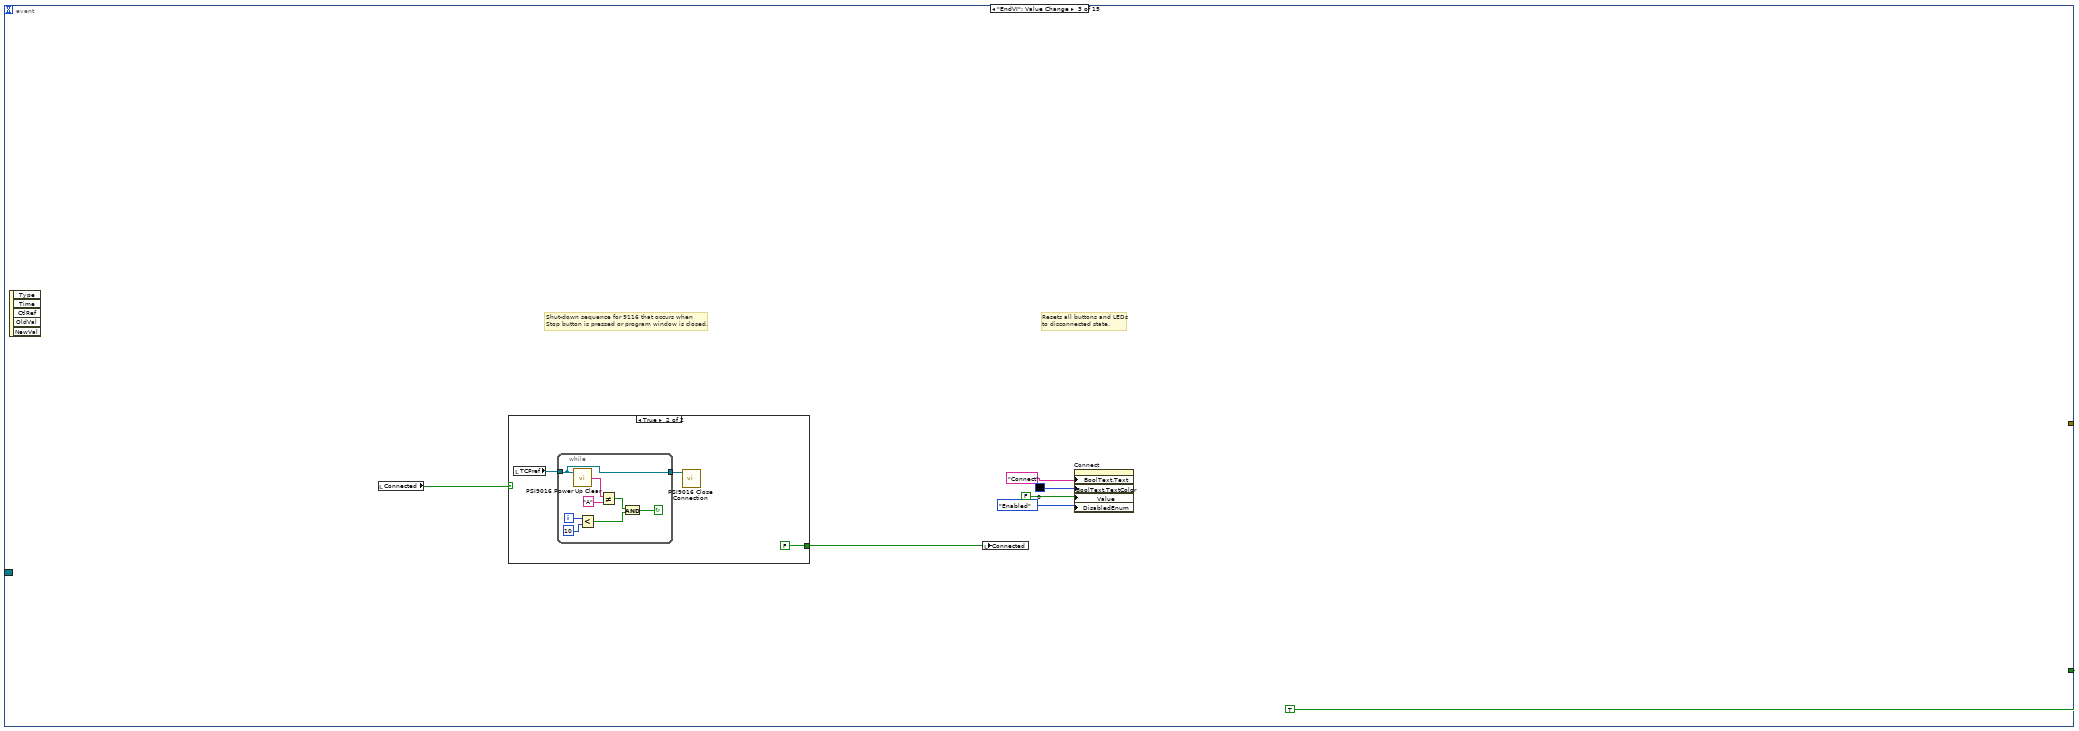
[diagram p6: hidden frame]
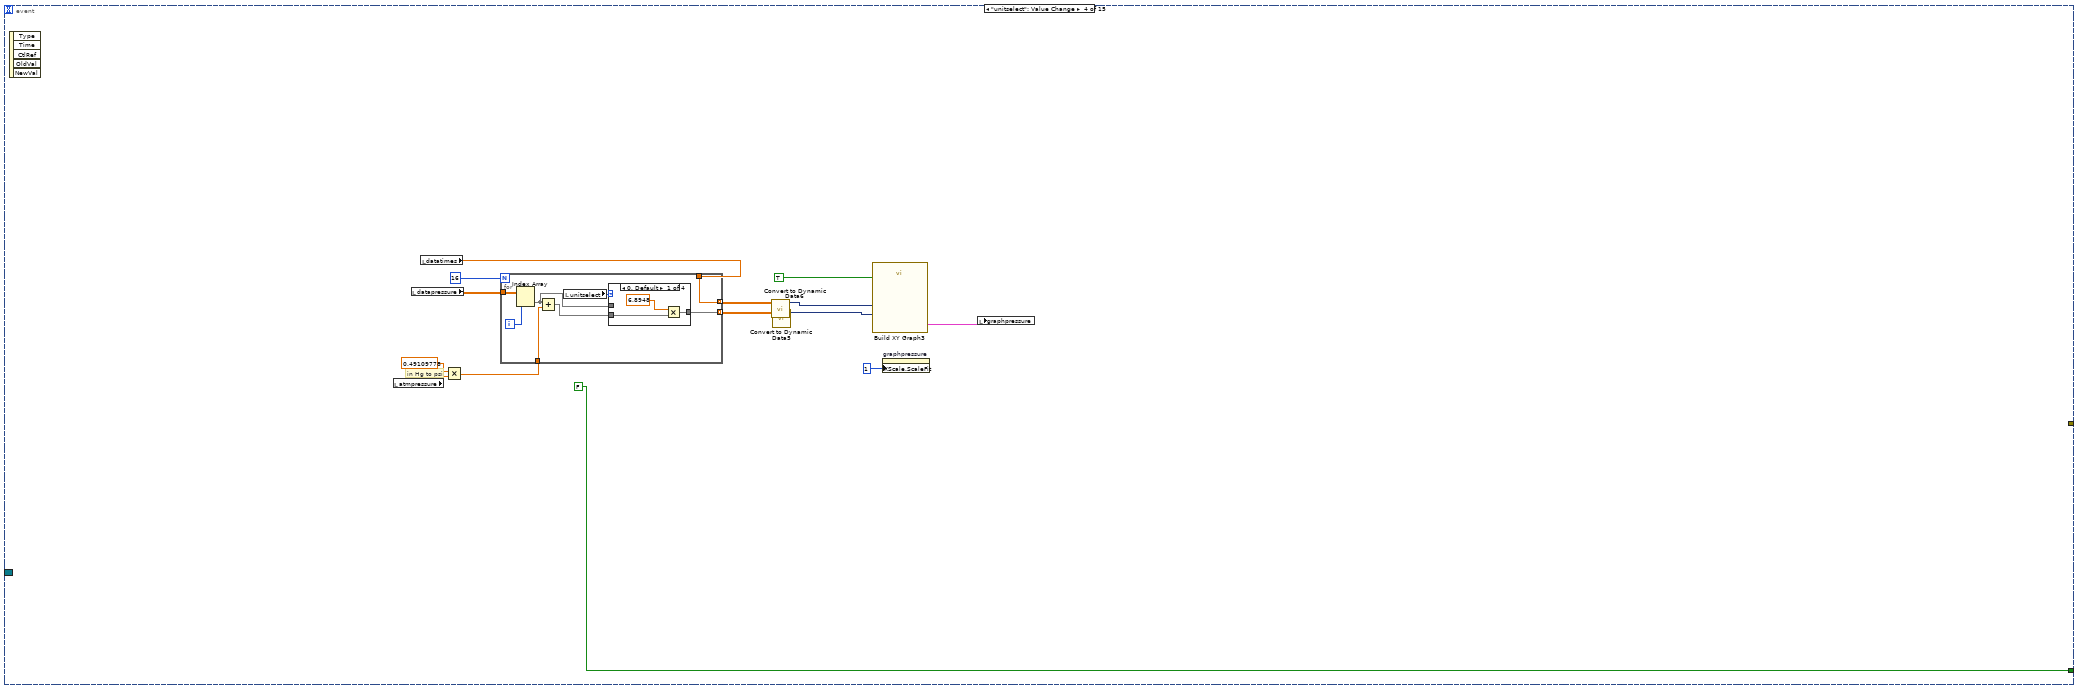
[diagram p8: hidden frame]
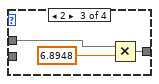
[diagram p10: hidden frame]
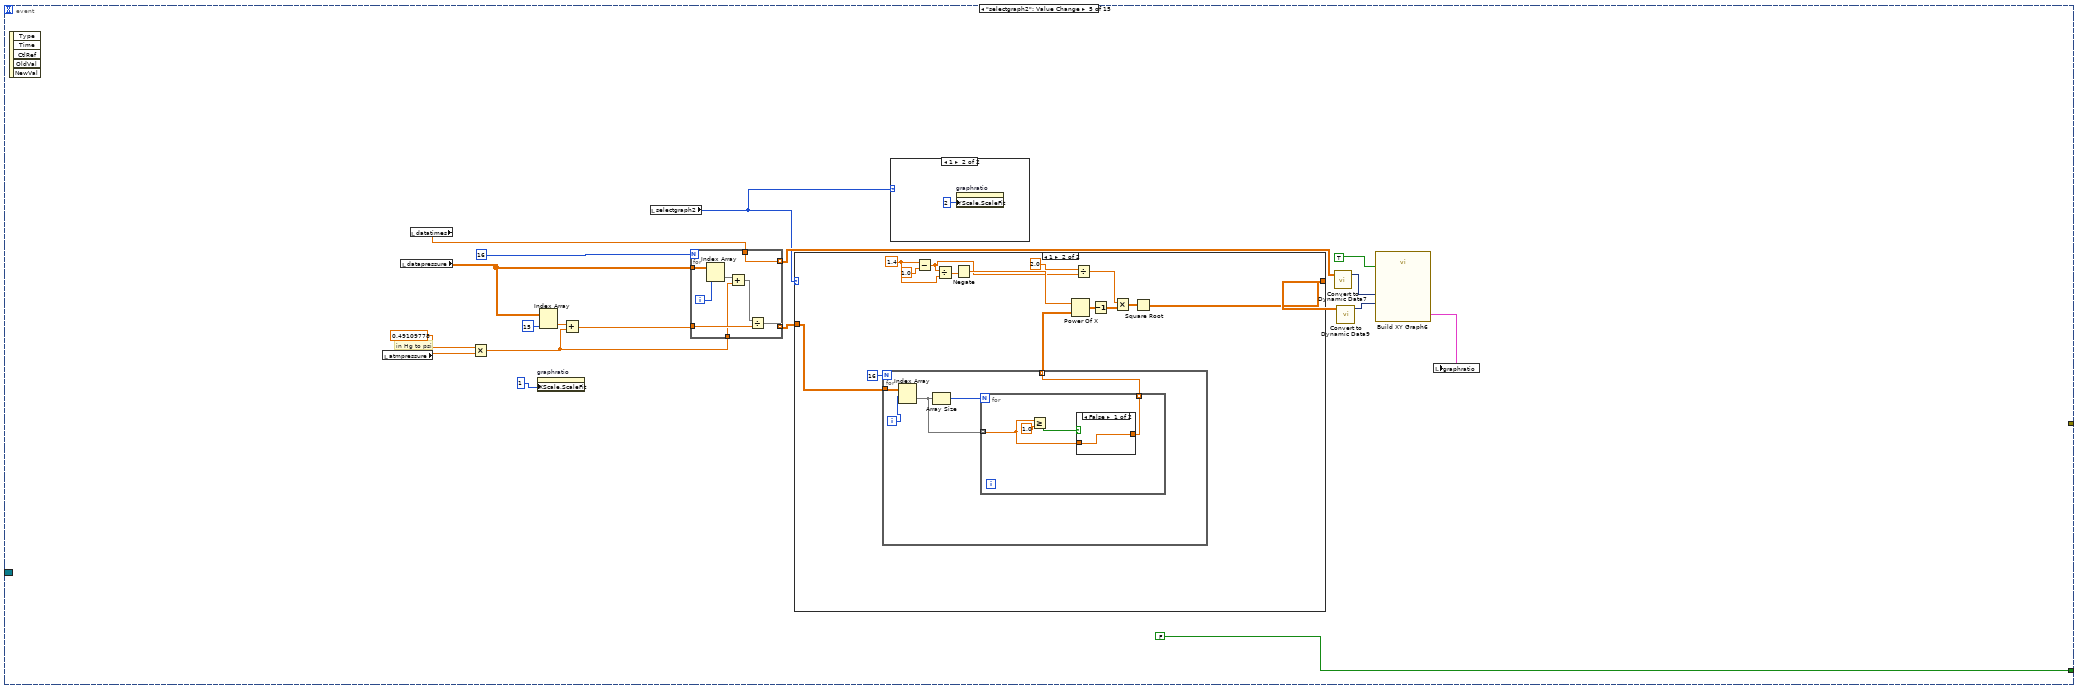
[diagram p12: hidden frame]
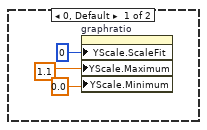
[diagram p13: hidden frame]
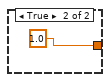
[diagram p15: hidden frame]
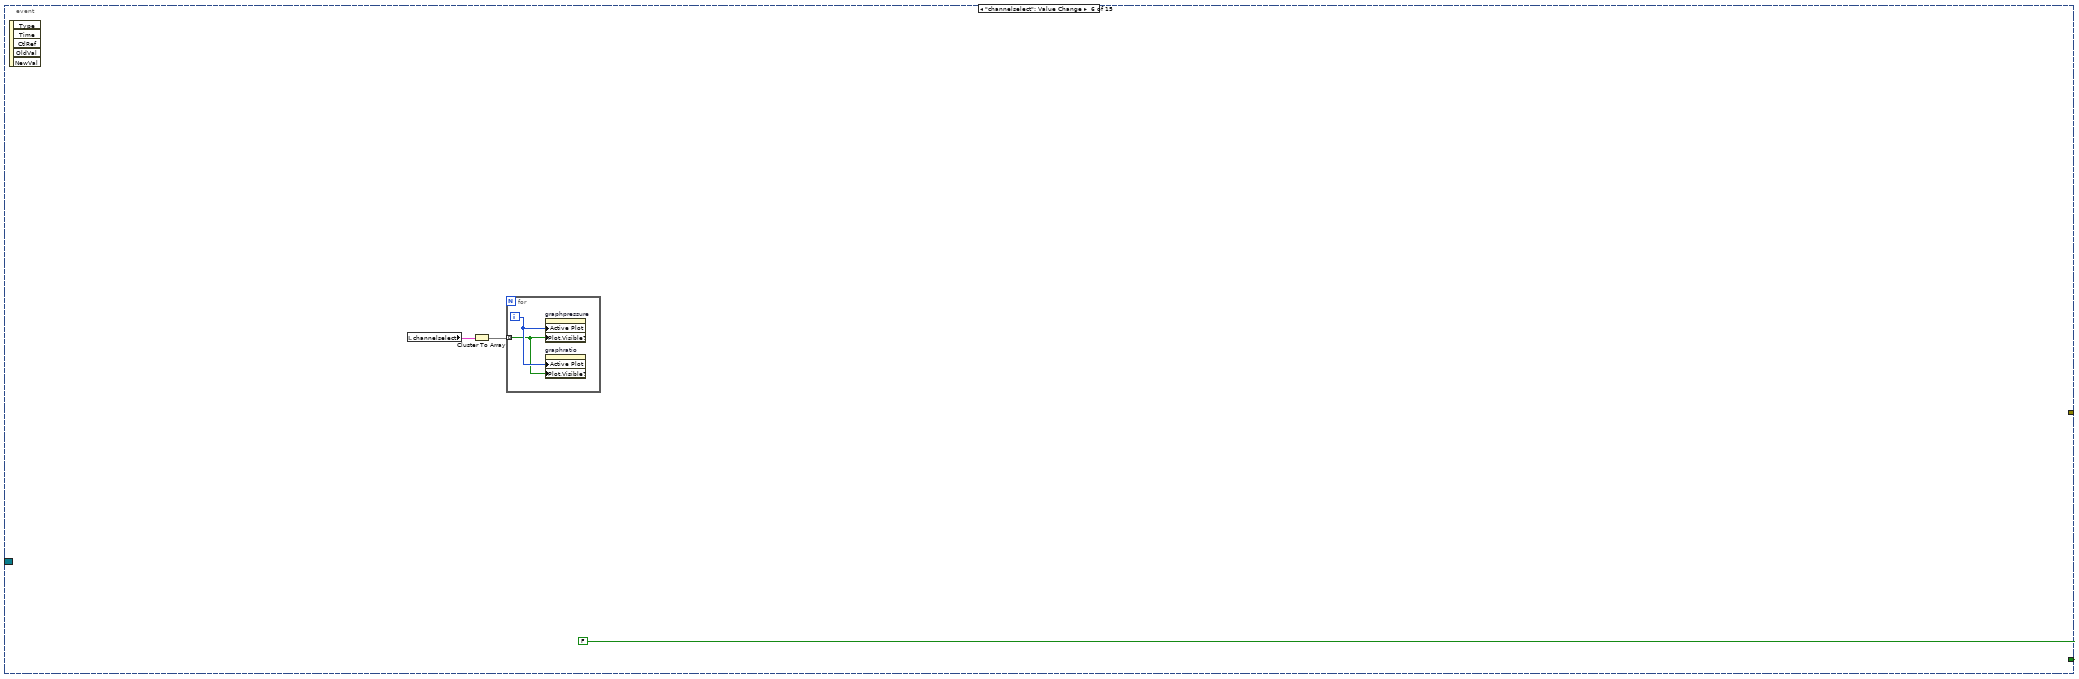
[diagram p16: hidden frame]
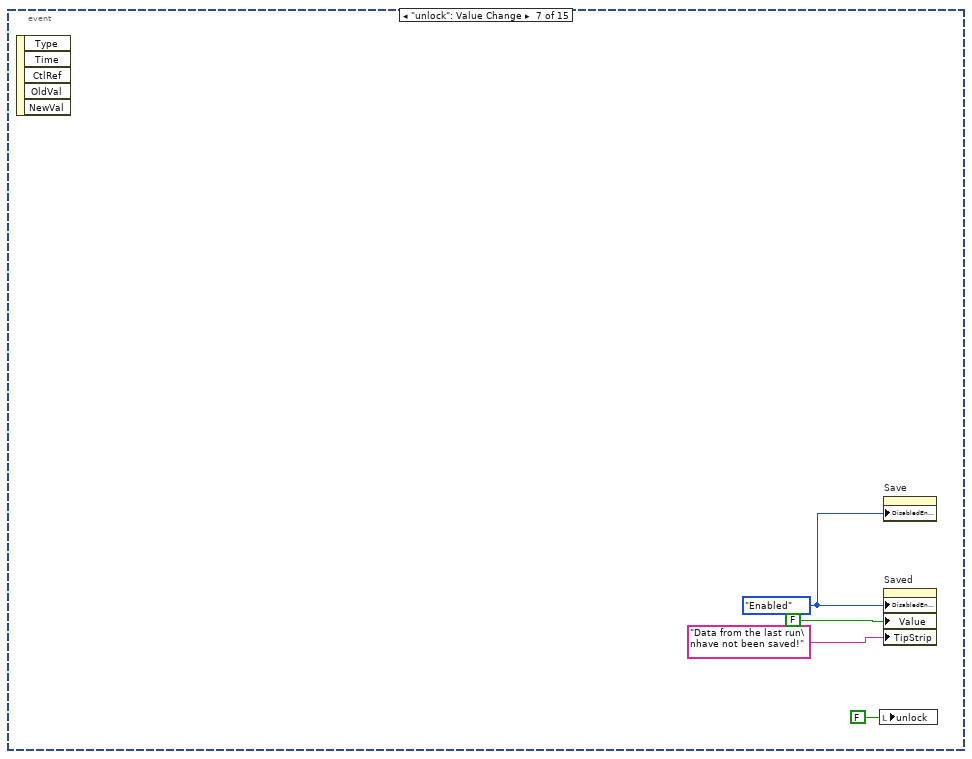
[diagram p17: hidden frame]
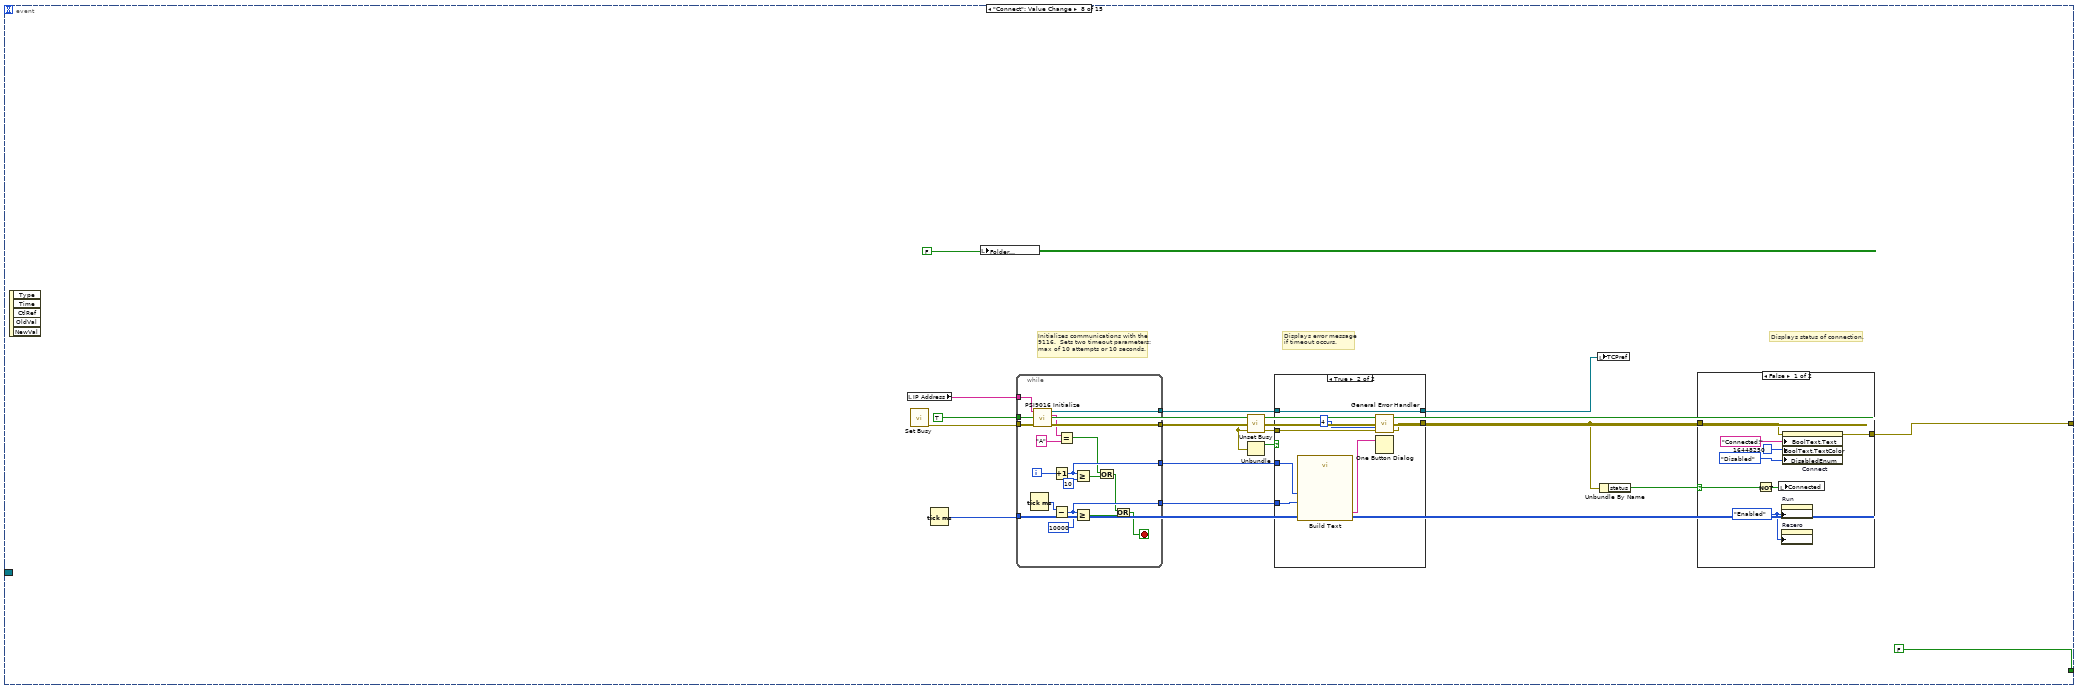
[diagram p18: hidden frame]
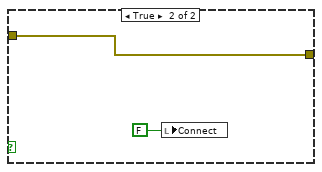
[diagram p19: hidden frame]
diagram:
  w1 = "" ("Load feedback")
  w3 = FALSE ("Dummy \nsave:")
  w11 = ""  # Initialize
  # "\"datum\" contains the last set\nof data polled from the 9116.\n\n\"data\" contains all samples\ncollected during a run sequence."
  # "Outputs/\nIndicators"
  # "Inputs"
  n1 = property on="graphratio" class="XYGraph (strict)"("YScale.ScaleFit"=u8 0 ("Y Scale.Scale Fit"), "YScale.Minimum"=0.0 ("Y Scale.Range:Minimum"), "YScale.Maximum"=1.1 ("Y Scale.Range:Maximum")) -> ()  [unwired: 2 in, 2 out]
  n2 = Create User Event(user event datatype=w11) -> (user event=w8:refnum<user-event>)  [unwired: 1 in, 1 out]
  n3 = register-events(w8) -> (reference out=w9:refnum<event-registration>, error out=w12:errorcluster)  [unwired: 2 in]
  n4 = String To Path(string=w1) -> (path=w2:path)
  n5 = property on="Load past data:" class="Path"("Value"=w2) -> ()  [unwired: 2 in, 2 out]
  n6 = Generate User Event(user event=w8, event data cluster="Initialization" ("event data"), error in=w12) -> (error out=w7:errorcluster)  [unwired: 1 in, 1 out]
  n7 = while {
    tunnel: w9 -> [w16]
    tunnel: w7 -> [_]
    stop <- w17 stop-if-true
    n8 = event shown="[12] \"Run\": Value Change" {
      selector: w16 -> [_ _ _ _ _ _ _ _ _ _ _ _ _ _ _]
      dyn-events: _ -> [_ _ _ _ _ _ _ _ _ _ _ _ _ _ _]
      timeout: 10000 -> [_ _ _ _ _ _ _ _ _ _ _ _ _ _ _]
      tunnel: [_ _ _ _ _ _ _ w161 w203 _ _ _ w278 _ _] -> w19
      tunnel: [FALSE ("Stop") _ TRUE ("Stop") FALSE ("Stop") FALSE ("Stop") FALSE ("Stop") _ FALSE ("Stop") FALSE ("Stop") FALSE ("Stop") _ _ FALSE ("Stop") _ FALSE ("Stop")] -> w17
      event User Event {
        w21 = T2."Disabled and Grayed Out" ("Disabled")
        w22 = FALSE ("stop")
        n9 = event-data() -> ()  [unwired: 1 in, 4 out]
        n10 = local read "channelselect"() -> (w25:T1)
        n11 = local read "unitselect"() -> (w24:u16)
        n12 = local write "EndVI"(w22) -> ()
        n13 = local write "Connected"(w22) -> ()
        n14 = local write "Connect"(w22) -> ()
        n15 = property on="Run" class="Bool (strict)"("DisabledEnum"=w21) -> ()  [unwired: 2 in, 2 out]
        n16 = property on="Saved" class="Bool (strict)"("DisabledEnum"=w21, "Value"=w22) -> ()  [unwired: 2 in, 2 out]
        n17 = property on="Save" class="Bool (strict)"("DisabledEnum"=w21) -> ()  [unwired: 2 in, 2 out]
        n18 = property on="Rezero" class="Bool"("DisabledEnum"=w21) -> ()  [unwired: 2 in, 2 out]
        n19 = property on="Runstop" class="Bool (strict)"("DisabledEnum"=w21) -> ()  [unwired: 2 in, 2 out]
        n20 = property on="channelselect" class="Clust (strict)"("Val(Sgnl)"=w25) -> ()  [unwired: 2 in, 2 out]
        n21 = property on="unitselect" class="Ring (strict)"("Val(Sgnl)"=w24) -> ()  [unwired: 2 in, 2 out]
      }
      event "Toggle 1-15": Value Change {
        n22 = event-data() -> ()  [unwired: 1 in, 5 out]
        n23 = case shown="True" "Toggle 1-15" {
          tunnel: ["Ones" "Zeros"] -> w27
          frame False {
          }
          frame True {
          }
        }
        n24 = Cluster To Array(cluster=w27) -> (array=w26:bool[])
        n25 = local write "channelselect"(w27) -> ()
        n26 = for {
          tunnel: w26 -> [w29] mode=indexing
          i -> [w30]
          n27 = property on="graphpressure" class="XYGraph (strict)"("Active Plot"=w30, "Plot.Visible?"=w29) -> ()  [unwired: 2 in, 2 out]
          n28 = property on="graphratio" class="XYGraph (strict)"("Active Plot"=w30, "Plot.Visible?"=w29) -> ()  [unwired: 2 in, 2 out]
        }
      }
      event "EndVI": Value Change {
        # "Resets all buttons and LEDs\nto disconnected state."
        # "Shut-down sequence for 9116 that occurs when \nStop button is pressed or program window is closed."
        n29 = event-data() -> ()  [unwired: 1 in, 5 out]
        n30 = local read "Connected"() -> (w39:bool)
        n31 = case shown="True" w39 {
          selector: w39 -> [w40 _]
          tunnel: [w40 FALSE] -> w38
          frame False {
          }
          frame True {
            n32 = local read "TCPref"() -> (w41:refnum<k5>)
            n33 = while {
              tunnel: [w49] -> w42
              tunnel: w41 -> [w49]
              i -> [w48]
              stop <- w44 continue-if-true
              n34 = call "PSI9016 Power Up Clear.vi"("TCP connection ref in"=w49) -> ("response"=w51:string)  [unwired: 2 in, 2 out]
              n35 = Less?(x=w48, y=10) -> (x < y?=w45:bool)
              n36 = Not Equal?(x=w51, y="A") -> (x != y?=w46:bool)
              n37 = And(x=w46, y=w45) -> (x .and. y?=w44:bool)
            }
            n38 = call "PSI9016 Close Connection.vi"("TCP connection ref in"=w42) -> ()  [unwired: 3 in, 1 out]
          }
        }
        n39 = local write "Connected"(w38) -> ()
        n40 = property on="Connect" class="Bool (strict)"("BoolText.Text"="Connect" ("Boolean Text.Text"), "BoolText.TextColor"=u32 0, "Value"=FALSE ("Connect"), "DisabledEnum"=T2."Enabled" ("Disabled")) -> ()  [unwired: 2 in, 2 out]
      }
      event "unitselect": Value Change {
        # "in Hg to psi"
        n41 = event-data() -> ()  [unwired: 1 in, 5 out]
        n42 = local read "atmpressure"() -> (w55:dbl)
        n43 = local read "datapressure"() -> (w52:dbl[][])
        n44 = local read "datatimes"() -> (w62:dbl[])
        n45 = Multiply(x=0.49109778, y=w55) -> (x*y=w57:dbl)
        n46 = for {
          N: 16 -> [_]
          tunnel: w52 -> [w73]
          tunnel: w57 -> [w72]
          tunnel: [w69] -> w59 mode=indexing
          tunnel: [w68] -> w61 mode=indexing
          tunnel: w62 -> [w68]
          i -> [w66]
          n47 = Index Array(array=w73, index (col)=w66) -> (element=w71:dbl[])  [unwired: 1 in]
          n48 = Add(x=w71, y=w72) -> (x+y=w70:dbl[])
          n49 = local read "unitselect"() -> (w67:u16)
          n50 = case shown="0, Default" w67 {
            tunnel: [w76 w77 w79 w81] -> w69
            tunnel: w71 -> [_ _ w78 w81]
            tunnel: w70 -> [w75 w77 _ _]
            frame 0, Default {
              n51 = Multiply(x=6.8948 ("y"), y=w75) -> (x*y=w76:dbl[])
            }
            frame 1 {
            }
            frame 2 {
              n52 = Multiply(x=w78, y=6.8948) -> (x*y=w79:dbl[])
            }
            frame 3 {
            }
          }
        }
        n53 = call "Convert to Dynamic Data6"("2D Array"=w61) -> ("Dynamic Data Type"=w63:dynamicdata)  [unwired: 3 in]
        n54 = call "Convert to Dynamic Data5"("2D Array"=w59) -> ("Dynamic Data Type"=w60:dynamicdata)  [unwired: 3 in]
        n55 = call "Build XY Graph3"("Reset"=TRUE, "Y Input"=w60, "X Input"=w63) -> ("XY Graph"=w64:cluster{"Y":dbl[], "Y":dbl[]}[])  [unwired: 7 in, 1 out]
        n56 = property on="graphpressure" class="XYGraph (strict)"("XScale.ScaleFit"=u8 1 ("X Scale.Scale Fit")) -> ()  [unwired: 2 in, 2 out]
        n57 = local write "graphpressure"(w64) -> ()
      }
      event "selectgraph2": Value Change {
        # "in Hg to psi"
        n58 = event-data() -> ()  [unwired: 1 in, 5 out]
        n59 = local read "atmpressure"() -> (w88:dbl)
        n60 = local read "datapressure"() -> (w85:dbl[][])
        n61 = local read "datatimes"() -> (w96:dbl[])
        n62 = Multiply(x=0.49109778, y=w88) -> (x*y=w90:dbl)
        n63 = property on="graphratio" class="XYGraph (strict)"("XScale.ScaleFit"=u8 1 ("X Scale.Scale Fit")) -> ()  [unwired: 2 in, 2 out]
        n64 = Index Array(array=w85, index (col)=15 ("disabled index (col)")) -> (element=w93:dbl[])  [unwired: 1 in]
        n65 = Add(x=w93, y=w90) -> (x+y=w92:dbl[])
        n66 = local read "selectgraph2"() -> (w82:u16)
        n67 = for {
          N: 16 -> [_]
          tunnel: w85 -> [w137]
          tunnel: w92 -> [w138]
          tunnel: w90 -> [w136]
          tunnel: [w131] -> w84 mode=indexing
          tunnel: [w133] -> w95 mode=indexing
          tunnel: w96 -> [w133]
          i -> [w132]
          n68 = Index Array(array=w137, index (col)=w132) -> (element=w135:dbl[])  [unwired: 1 in]
          n69 = Add(x=w135, y=w136) -> (x+y=w134:dbl[])
          n70 = Divide(x=w134, y=w138) -> (x/y=w131:dbl[])
        }
        n71 = case shown="1" w82 {
          tunnel: w84 -> [w105 w110]
          tunnel: [w105 w107] -> w83
          frame 0, Default {
          }
          frame 1 {
            w118 = 1.4
            n72 = for {
              N: 16 -> [_]
              tunnel: w110 -> [w124]
              tunnel: [w120] -> w109 mode=indexing
              i -> [w121]
              n73 = Index Array(array=w124, index (row)=w121) -> (element=w122:dbl[])  [unwired: 1 in]
              n74 = Array Size(array=w122) -> (size(s)=w123:i32)
              n75 = for {
                N: w123 -> [_]
                tunnel: w122 -> [w126] mode=indexing
                tunnel: [w125] -> w120 mode=indexing
                n76 = Greater Or Equal?(x=w126, y=1.0) -> (x >= y?=w127:bool)
                n77 = case shown="False" w127 {
                  tunnel: w126 -> [w129 _]
                  tunnel: [w129 1.0] -> w125
                  frame False {
                  }
                  frame True {
                  }
                }
              }
            }
            n78 = Subtract(x=w118, y=1.0) -> (x-y=w114:dbl)
            n79 = Divide(x=w114, y=w118) -> (x/y=w117:dbl)
            n80 = Negate(x=w117) -> (-x=w116:dbl)
            n81 = Power Of X(1:w109, 2:w116) -> (0:w106:dbl[][])
            n82 = Divide(x=2.0, y=w114) -> (x/y=w112:dbl)
            n83 = Decrement(x=w106) -> (x-1=w115:dbl[][])
            n84 = Multiply(x=w112, y=w115) -> (x*y=w111:dbl[][])
            n85 = Square Root(x=w111) -> (sqrt(x)=w107:dbl[][])
          }
        }
        n86 = case shown="1" w82 {
          frame 0, Default {
            n87 = property on="graphratio" class="XYGraph (strict)"("YScale.ScaleFit"=u8 0 ("Y Scale.Scale Fit"), "YScale.Maximum"=1.1, "YScale.Minimum"=0.0 ("Y Scale.Range:Minimum")) -> ()  [unwired: 2 in, 2 out]
          }
          frame 1 {
            n88 = property on="graphratio" class="XYGraph (strict)"("YScale.ScaleFit"=u8 2 ("Y Scale.Scale Fit")) -> ()  [unwired: 2 in, 2 out]
          }
        }
        n89 = call "Convert to Dynamic Data7"("2D Array"=w95) -> ("Dynamic Data Type"=w97:dynamicdata)  [unwired: 3 in]
        n90 = call "Convert to Dynamic Data9"("2D Array"=w83) -> ("Dynamic Data Type"=w94:dynamicdata)  [unwired: 3 in]
        n91 = call "Build XY Graph6"("Reset"=TRUE, "Y Input"=w94, "X Input"=w97) -> ("XY Graph"=w98:cluster{"Y":dbl[], "Y":dbl[]}[])  [unwired: 7 in, 1 out]
        n92 = local write "graphratio"(w98) -> ()
      }
      event "channelselect": Value Change {
        n93 = event-data() -> ()  [unwired: 1 in, 5 out]
        n94 = local read "channelselect"() -> (w140:T1)
        n95 = Cluster To Array(cluster=w140) -> (array=w141:bool[])
        n96 = for {
          tunnel: w141 -> [w142] mode=indexing
          i -> [w143]
          n97 = property on="graphpressure" class="XYGraph (strict)"("Active Plot"=w143, "Plot.Visible?"=w142) -> ()  [unwired: 2 in, 2 out]
          n98 = property on="graphratio" class="XYGraph (strict)"("Active Plot"=w143, "Plot.Visible?"=w142) -> ()  [unwired: 2 in, 2 out]
        }
      }
      event "unlock": Value Change {
        w145 = T2."Enabled" ("Disabled")
        n99 = event-data() -> ()  [unwired: 1 in, 5 out]
        n100 = local write "unlock"(FALSE ("unlock")) -> ()
        n101 = property on="Save" class="Bool (strict)"("DisabledEnum"=w145) -> ()  [unwired: 2 in, 2 out]
        n102 = property on="Saved" class="Bool (strict)"("DisabledEnum"=w145, "Value"=FALSE ("Saved"), "TipStrip"="Data from the last run\nhave not been saved!" ("Tip Strip")) -> ()  [unwired: 2 in, 2 out]
      }
      event "Connect": Value Change {
        # "Displays status of connection."
        # "Displays error message\nif timeout occurs."
        # "Initializes communications with the\n9116.  Sets two timeout parameters:\nmax of 10 attempts or 10 seconds."
        n103 = event-data() -> ()  [unwired: 1 in, 5 out]
        n104 = local read "IP Address"() -> (w162:string)
        n105 = call <vilib>:"Set Busy.vi"() -> ("error out"=w160:errorcluster)  [unwired: 10 in, 1 out]
        n106 = Tick Count (ms)() -> (millisecond timer value=w157:u32)
        n107 = local write "Folder \nchange:"(FALSE) -> ()
        n108 = while {
          tunnel: w162 -> [w201]
          tunnel: [w185] -> w159
          tunnel: TRUE ("Power Up Clear") -> [w200]
          tunnel: [w184] -> w153
          tunnel: w160 -> [w196]
          tunnel: w157 -> [w193]
          tunnel: [w191] -> w156
          tunnel: [w190] -> w155
          i -> [w197]
          stop <- w186 stop-if-true
          n109 = Tick Count (ms)() -> (millisecond timer value=w194:u32)
          n110 = call "PSI9016 Initialize.vi"("IP Address"=w201, "power up clear"=w200, "error in (no error)"=w196) -> ("TCP Connection Ref out"=w185:refnum<k5>, "Power Up Clear Response"=w199:string, "error out"=w184:errorcluster)  [unwired: 1 out]
          n111 = Increment(x=w197) -> (x+1=w191:i32)
          n112 = Subtract(x=w194, y=w193) -> (x-y=w190:u32)
          n113 = Equal?(x=w199, y="A") -> (x = y?=w183:bool)
          n114 = Greater Or Equal?(x=w191, y=10) -> (x >= y?=w189:bool)
          n115 = Greater Or Equal?(x=w190, y=u32 10000) -> (x >= y?=w187:bool)
          n116 = Or(x=w183, y=w189) -> (x .or. y?=w188:bool)
          n117 = Or(x=w188, y=w187) -> (x .or. y?=w186:bool)
        }
        n118 = call <vilib>:"Unset Busy.vi"("error in (no error)"=w153) -> ("error out"=w158:errorcluster)  [unwired: 10 in]
        n119 = Unbundle(w153) -> ("status"=w154:bool)  [unwired: 2 out]
        n120 = case shown="True" w154 {
          tunnel: w159 -> [w175 w181]
          tunnel: [w175 w181] -> w151
          tunnel: w158 -> [w174 w179]
          tunnel: [w174 w180] -> w149
          tunnel: w156 -> [_ w178]
          tunnel: w155 -> [_ w177]
          frame False {
          }
          frame True {
            n121 = call "Build Text"("attempts"=w178, "time"=w177) -> ("Result"=w176:string)  [unwired: 12 in, 1 out]
            n122 = call <vilib>:"General Error Handler.vi"("type of dialog (OK msg:1)"=4, "error in (no error)"=w179) -> ("error out"=w180:errorcluster)  [unwired: 9 in, 4 out]
            n123 = One Button Dialog(message=w176) -> ()  [unwired: 1 in, 1 out]
          }
        }
        n124 = local write "TCPref"(w151) -> ()
        n125 = Unbundle By Name(w149) -> ("status"=w150:bool)
        n126 = case shown="False" w150 {
          selector: w150 -> [w165 _]
          tunnel: w149 -> [w167 w173]
          tunnel: [w166 w173] -> w161
          frame False {
            w164 = T2."Enabled" ("Disabled")
            n127 = Not(x=w165) -> (.not. x?=w169:bool)
            n128 = local write "Connected"(w169) -> ()
            n129 = property on="Run" class="Bool (strict)"("DisabledEnum"=w164) -> ()  [unwired: 2 in, 2 out]
            n130 = property on="Rezero" class="Bool"("DisabledEnum"=w164) -> ()  [unwired: 2 in, 2 out]
            n131 = property on="Connect" class="Bool (strict)"(error in=w167, "BoolText.Text"="Connected!" ("Boolean Text.Text"), "BoolText.TextColor"=u32 16448250, "DisabledEnum"=T2."Disabled" ("Disabled")) -> (error out=w166:errorcluster)  [unwired: 1 in, 1 out]
          }
          frame True {
            n132 = local write "Connect"(FALSE ("Connect")) -> ()
          }
        }
      }
      event "Rezero": Value Change {
        n133 = event-data() -> ()  [unwired: 1 in, 5 out]
        n134 = call "Display Message to User"() -> ("Rezero"=w205:bool)  [unwired: 10 in, 1 out]
        n135 = local write "Folder \nchange:"(FALSE) -> ()
        n136 = local read "TCPref"() -> (w204:refnum<k5>)
        n137 = case shown="False" w205 {
          tunnel: w204 -> [_ w207]
          tunnel: [_ w210] -> w203
          frame False {
          }
          frame True {
            n138 = call <vilib>:"Set Busy.vi"() -> ("error out"=w209:errorcluster)  [unwired: 10 in, 1 out]
            n139 = call "PSI9016 ReZero.vi"("error in (no error)"=w209, "TCP connection ref in"=w207) -> ("error out"=w211:errorcluster, "rezero counts"=w208:dbl[])  [unwired: 1 in, 1 out]
            n140 = local write "Rezero Values"(w208) -> ()
            n141 = call <vilib>:"Unset Busy.vi"("error in (no error)"=w211) -> ("error out"=w210:errorcluster)  [unwired: 10 in]
          }
        }
      }
      event "Save": Value Change {
        n142 = event-data() -> ()  [unwired: 1 in, 5 out]
        n143 = flat-sequence {
          frame #0 {
            n144 = local read "Dummy \nsave:"() -> (w213:bool)
            n145 = case shown="True" w213 {
              frame False {
              }
              frame True {
                n146 = local read "Saved file:"() -> (w215:string)
                n147 = local read "Folder path:"() -> (w216:path)
                n148 = Build Path(base path=w216, name or relative path=w215) -> (appended path=w214:path)
                n149 = Delete(path (use dialog)=w214) -> ()  [unwired: 4 in, 3 out]
              }
            }
          }
          frame #1 {
            n150 = local read "datapressure"() -> (w222:dbl[][])
            n151 = local read "atmpressure"() -> (w223:dbl)
            n152 = local read "Folder path:"() -> (w218:path)
            n153 = local read "datatimes"() -> (w220:dbl[])
            n154 = local read "File prefix:"() -> (w221:string)
            n155 = local read "run time"() -> (w219:timestamp)
            n156 = call "save_p_data.vi"("File prefix:"=w221, "run time"=w219, "Folder path:"=w218, "datapressure"=w222, "atmpressure"=w223, "datatimes"=w220) -> ("Saved file:"=w224:string, "Output folder:"=w217:path, "Folder \nchanged:"=w225:bool)  [unwired: 11 in]
            n157 = local write "Folder path:"(w217) -> ()
            n158 = local write "Saved file:"(w224) -> ()
            n159 = local write "Folder \nchange:"(w225) -> ()
          }
          frame #2 {
            w228 = FALSE ("Save")
            n160 = property on="Saved" class="Bool (strict)"("Value"=TRUE ("Saved"), "TipStrip"="Data from the last run\nhave been saved." ("Tip Strip")) -> ()  [unwired: 2 in, 2 out]
            n161 = local write "Save"(w228) -> ()
            n162 = local write "Dummy \nsave:"(w228) -> ()
          }
        }
      }
      event "Folder path:": Value Change {
        n163 = event-data() -> ()  [unwired: 1 in, 6 out]
        n164 = local read "Folder path:"() -> (w229:path)
        n165 = property on="Load past data:" class="Path"("StartPath"=w229) -> ()  [unwired: 2 in, 2 out]
      }
      event "Load past data:": Value Change {
        n166 = event-data() -> ()  [unwired: 1 in, 6 out]
        n167 = local read "Load past data:"() -> (w230:path)
        n168 = Path To String(path=w230) -> (string=w237:string)
        n169 = String Length(string=w237) -> (length=w235:i32)
        n170 = Subtract(x=w235, y=3) -> (x-y=w236:i32)
        n171 = String Subset(string=w237, offset (0)=w236) -> (substring=w233:string)  [unwired: 1 in]
        n172 = Equal?(x=w233, y="csv") -> (x = y?=w231:bool)
        n173 = case shown="True" w231 {
          tunnel: w230 -> [_ w245]
          frame False {
            n174 = local write "Load feedback"("Not a .csv, try again.") -> ()
          }
          frame True {
            n175 = local write "Load feedback"("") -> ()
            n176 = Path To String(path=w245) -> (string=w243:string)
            n177 = call-poly <vilib>:"Read From Spreadsheet File.vi"("number of rows (all:-1)"=2, "file path (dialog if empty)"=w245) -> ("all rows"=w258:string[][])  [unwired: 5 in, 4 out]
            n178 = call "Read From Measurement File"("Filename"=w245) -> ("Signals"=w270:dynamicdata)  [unwired: 5 in, 5 out]
            n179 = Reverse String(1:w243) -> (0:w242:string)
            n180 = Index Array(array=w258, index (row)=1) -> (element=w256:string[])  [unwired: 1 in]
            n181 = Array of Strings to Path(0:w256) -> (2:w255:path)  [unwired: 1 in]
            n182 = Search/Split String(string=w242, search string/char (-)="\\") -> (match + rest of string=w241:string)  [unwired: 1 in, 2 out]
            n183 = call "Convert from Dynamic Data"("Dynamic Data Type"=w270) -> ("Array"=w269:dbl[][])  [unwired: 3 in]
            n184 = Path To String(path=w255) -> (string=w254:string)
            n185 = Reverse String(1:w241) -> (0:w240:string)
            n186 = Transpose 2D Array(2D array=w269) -> (transposed array=w267:dbl[][])
            n187 = Array Subset(array=w267, index (row)=1 ("index")) -> (w265:dbl[][])  [unwired: 3 in]
            n188 = Scan From String(format string="%s %s %f", input string=w254) -> (output 3=w250:dbl)  [unwired: 7 in, 3 out]
            n189 = String To Path(string=w240) -> (path=w239:path)
            n190 = Transpose 2D Array(2D array=w265) -> (transposed array=w251:dbl[][])
            n191 = Index Array(array=w267, index (row)=0 ("index")) -> (element=w264:dbl[])  [unwired: 1 in]
            n192 = property on="Load past data:" class="Path"("StartPath"=w239) -> ()  [unwired: 2 in, 2 out]
            n193 = Divide(x=w251, y=6894.8) -> (x/y=w249:dbl[][])
            n194 = Multiply(x=0.49109778, y=w250) -> (x*y=w247:dbl)
            n195 = Subtract(x=w249, y=w247) -> (x-y=w248:dbl[][])
            n196 = local write "datapressure"(w248) -> ()
            n197 = local write "datatimes"(w264) -> ()
            n198 = call "Convert to Dynamic Data4"("Array"=w264) -> ("Dynamic Data Type"=w263:dynamicdata)  [unwired: 3 in]
            n199 = call "Convert to Dynamic Data8"("2D Array"=w248) -> ("Dynamic Data Type"=w262:dynamicdata)  [unwired: 3 in]
            n200 = call "Build XY Graph4"("Reset"=TRUE, "Y Input"=w262, "X Input"=w263) -> ("XY Graph"=w261:cluster{"Y":dbl[], "Y":dbl[]}[])  [unwired: 7 in, 1 out]
            n201 = flat-sequence {
              tunnel: w261 -> [w272]
              frame #0 {
                n202 = local write "graphpressure"(w272) -> ()
              }
              frame #1 {
                n203 = local read "selectgraph2"() -> (w273:u16)
                n204 = local read "unitselect"() -> (w274:u16)
                n205 = property on="selectgraph2" class="Ring (strict)"("Val(Sgnl)"=w273) -> ()  [unwired: 2 in, 2 out]
                n206 = property on="unitselect" class="Ring (strict)"("Val(Sgnl)"=w274) -> ()  [unwired: 2 in, 2 out]
              }
              frame #2 {
                n207 = local read "selectgraph2"() -> (w275:u16)
                n208 = local read "unitselect"() -> (w276:u16)
                n209 = property on="selectgraph2" class="Ring (strict)"("Val(Sgnl)"=w275) -> ()  [unwired: 2 in, 2 out]
                n210 = property on="unitselect" class="Ring (strict)"("Val(Sgnl)"=w276) -> ()  [unwired: 2 in, 2 out]
              }
            }
          }
        }
      }
      event "Run": Value Change {
        n211 = event-data() -> ()  [unwired: 1 in, 5 out]
        n212 = flat-sequence {
          tunnel: [w285] -> w277
          tunnel: [w448] -> w278
          tunnel: w277 -> [w448]
          frame #0 {
            w283 = "" ("Load feedback")
            # "in Hg to psi"
            n213 = String To Path(string=w283) -> (path=w282:path)
            n214 = local write "Load feedback"(w283) -> ()
            n215 = property on="Load past data:" class="Path"("Value"=w282) -> ()  [unwired: 2 in, 2 out]
            n216 = local write "Dummy \nsave:"(FALSE ("Dummy \nsave:")) -> ()
            n217 = flat-sequence {
              tunnel: [w317] -> w289
              tunnel: [w316] -> w288
              tunnel: [w315] -> w287
              tunnel: [w314] -> w286
              frame #0 {
                w313 = T2."Disabled and Grayed Out" ("Disabled")
                w324 = 0.0
                n218 = local read "timeinterval"() -> (w330:i32)
                n219 = local read "timetotal"() -> (w329:dbl)
                n220 = local read "TCPref"() -> (w321:refnum<k5>)
                n221 = call <vilib>:"Set Busy.vi"("disable click? (T)"=FALSE) -> ()  [unwired: 9 in, 2 out]
                n222 = Initialize Array(w324, 16 ("dimension size")) -> (w327:dbl[])
                n223 = Get Date/Time In Seconds() -> (seconds since 1Jan1904=→"run time":timestamp)
                n224 = Generate Occurrence() -> (w314:refnum<k4>)
                n225 = call "PSI9016 Configure Host Delivery Stream.vi"("TCP connection ref in"=w321, "per (100)"=w330, "num (0)"=i8 0) -> ("error out"=w328:errorcluster)  [unwired: 10 in, 2 out]
                n226 = local write "Running"(TRUE ("Running")) -> ()
                n227 = local write "datumpressure"(w327) -> ()
                n228 = local write "datumtime"(w324) -> ()
                n229 = property on="Run" class="Bool (strict)"("DisabledEnum"=T2."Disabled" ("Disabled")) -> ()  [unwired: 2 in, 2 out]
                n230 = property on="Runstop" class="Bool (strict)"("DisabledEnum"=T2."Enabled" ("Disabled")) -> ()  [unwired: 2 in, 2 out]
                n231 = property on="Runstop" class="Bool (strict)"("Visible"=TRUE) -> ()  [unwired: 2 in, 2 out]
                n232 = property on="graphpressure" class="XYGraph (strict)"("XScale.Maximum"=w329, "XScale.Minimum"=w324) -> ()  [unwired: 2 in, 2 out]
                n233 = property on="graphratio" class="XYGraph (strict)"("XScale.Maximum"=w329, "XScale.Minimum"=w324) -> ()  [unwired: 2 in, 2 out]
                n234 = call "PSI9016 Start Stream.vi"("error in (no error)"=w328, "TCP connection ref in"=w321) -> ("number of packets"=w316:i32, "error out"=w315:errorcluster, "TCP connection ref out"=w317:refnum<k5>)  [unwired: 2 in, 1 out]
                n235 = property on="channelselect" class="Clust (strict)"("DisabledEnum"=w313) -> ()  [unwired: 2 in, 2 out]
                n236 = property on="Toggle 1-15" class="Bool (strict)"("DisabledEnum"=w313) -> ()  [unwired: 2 in, 2 out]
                n237 = property on="unitselect" class="Ring (strict)"("DisabledEnum"=w313) -> ()  [unwired: 2 in, 2 out]
                n238 = property on="selectgraph2" class="Ring (strict)"("DisabledEnum"=w313) -> ()  [unwired: 2 in, 2 out]
                n239 = property on="EndVI" class="Bool (strict)"("DisabledEnum"=w313) -> ()  [unwired: 2 in, 2 out]
                n240 = property on="Open save folder" class="Bool (strict)"("DisabledEnum"=w313) -> ()  [unwired: 2 in, 2 out]
                n241 = property on="unlock" class="Bool (strict)"("DisabledEnum"=w313) -> ()  [unwired: 2 in, 2 out]
                n242 = property on="Load past data:" class="Path"("DisabledEnum"=w313) -> ()  [unwired: 2 in, 2 out]
                n243 = property on="Folder path:" class="Path"("DisabledEnum"=w313) -> ()  [unwired: 2 in, 2 out]
                n244 = property on="Rezero" class="Bool"("DisabledEnum"=w313) -> ()  [unwired: 2 in, 2 out]
              }
            }
            n245 = local write "Folder \nchange:"(FALSE) -> ()
            n246 = Wait on Occurrence(2:w286) -> (0:w301:bool)  [unwired: 2 in]
            n247 = local read "atmpressure"() -> (w298:dbl)
            n248 = local read "selectgraph2"() -> (w311:u16)
            n249 = local read "unitselect"() -> (w309:u16)
            n250 = Multiply(x=0.49109778, y=w298) -> (x*y=w300:dbl)
            n251 = while {
              tunnel: w300 -> [w350]
              tunnel: w301 -> [_]
              tunnel: [T2."Enabled" ("Disabled")] -> w280
              tunnel: [FALSE ("status")] -> w305
              tunnel: [w339] -> w304
              tunnel: [TRUE ("status")] -> w308
              tunnel: [T2."Disabled and Grayed Out" ("Disabled")] -> w307
              tunnel: w309 -> [w339]
              tunnel: w311 -> [w332]
              tunnel: [w332] -> w312
              i -> [w353]
              stop <- w362 continue-if-true
              n252 = local read "datumpressure"() -> (w361:dbl[])
              n253 = local read "datumtime"() -> (w347:dbl)
              n254 = Wait (ms)(milliseconds to wait=u32 25) -> ()  [unwired: 1 out]
              n255 = local read "Running"() -> (w362:bool)
              n256 = Index Array(array=w361, index=15 ("disabled index (col)")) -> (element=w358:dbl)
              n257 = Add(x=w358, y=w350) -> (x+y=w359:dbl)
              n258 = for {
                N: 16 -> [_]
                tunnel: w361 -> [w377]
                tunnel: w359 -> [w378]
                tunnel: w350 -> [w376]
                tunnel: [w372] -> w356 mode=indexing
                tunnel: [w367] -> w338 mode=indexing
                tunnel: [w371] -> w348 mode=indexing
                tunnel: w347 -> [w371]
                tunnel: w339 -> [w370]
                tunnel: w332 -> [w369]
                tunnel: [w368] -> w333 mode=indexing
                i -> [w373]
                n259 = Index Array(array=w377, index=w373) -> (element=w375:dbl)
                n260 = Add(x=w375, y=w376) -> (x+y=w374:dbl)
                n261 = Divide(x=w374, y=w378) -> (x/y=w367:dbl)
                n262 = case shown="0, Default" w370 {
                  tunnel: [w384 w385 w387 w389] -> w372
                  tunnel: w375 -> [_ _ w386 w389]
                  tunnel: w374 -> [w383 w385 _ _]
                  frame 0, Default {
                    n263 = Multiply(x=6.8948 ("y"), y=w383) -> (x*y=w384:dbl)
                  }
                  frame 1 {
                  }
                  frame 2 {
                    n264 = Multiply(x=w386, y=6.8948) -> (x*y=w387:dbl)
                  }
                  frame 3 {
                  }
                }
                n265 = case shown="1" w369 {
                  tunnel: [w379 w381] -> w368
                  tunnel: w367 -> [w379 w380]
                  frame 0, Default {
                  }
                  frame 1 {
                    n266 = call "p_p0.vi"("p/p0"=w380) -> ("M"=w381:dbl)
                  }
                }
              }
              n267 = local read "Mach_Chan_Select"() -> (w335:i16)
              n268 = Decrement(x=w335) -> (x-1=w334:i16)
              n269 = Index Array(array=w338, index=w334) -> (element=w337:dbl)
              n270 = call "p_p0.vi"("p/p0"=w337) -> ("M"=w336:dbl)
              n271 = local write "Chan_Mach"(w336) -> ()
              n272 = call "Convert to Dynamic Data2"("Array"=w333) -> ("Dynamic Data Type"=w354:dynamicdata)  [unwired: 3 in]
              n273 = call "Convert to Dynamic Data"("Array"=w356) -> ("Dynamic Data Type"=w355:dynamicdata)  [unwired: 3 in]
              n274 = call "Convert to Dynamic Data3"("Array"=w348) -> ("Dynamic Data Type"=w346:dynamicdata)  [unwired: 3 in]
              n275 = Equal?(x=w353, y=0) -> (x = y?=w351:bool)
              n276 = call "Build XY Graph"("Reset"=w351, "Y Input"=w355, "X Input"=w346) -> ("XY Graph"=w344:cluster{"Y":dbl[], "Y":dbl[]}[])  [unwired: 7 in, 1 out]
              n277 = call "Build XY Graph2"("Reset"=w351, "Y Input"=w354, "X Input"=w346) -> ("XY Graph"=w345:cluster{"Y":dbl[], "Y":dbl[]}[])  [unwired: 7 in, 1 out]
              n278 = local write "graphpressure"(w344) -> ()
              n279 = local write "graphratio"(w345) -> ()
              n280 = case shown="1" w332 {
                frame 0, Default {
                  n281 = property on="graphratio" class="XYGraph (strict)"("YScale.ScaleFit"=u8 0 ("Y Scale.Scale Fit"), "YScale.Maximum"=1.1, "YScale.Minimum"=0.0 ("Y Scale.Range:Minimum")) -> ()  [unwired: 2 in, 2 out]
                }
                frame 1 {
                  n282 = property on="graphratio" class="XYGraph (strict)"("YScale.ScaleFit"=u8 2 ("Y Scale.Scale Fit")) -> ()  [unwired: 2 in, 2 out]
                }
              }
            }
            n283 = local read "timetotal"() -> (w294:dbl)
            n284 = Tick Count (ms)() -> (millisecond timer value=w293:u32)
            n285 = Equal To 0?(x=w288) -> (x = 0?=w292:bool)
            n286 = while {
              shift-left: 0 -> [w422]
              shift-right: [w420] -> _
              tunnel: w289 -> [w394]
              tunnel: w292 -> [w426]
              shift-left: w288 -> [w424]
              shift-right: [w423] -> _
              tunnel: [w394] -> w290
              tunnel: w293 -> [w417]
              tunnel: w294 -> [w416]
              tunnel: w287 -> [w413]
              tunnel: [w412] -> w295
              tunnel: [w390] -> w302
              shift-right: [w409] -> w281
              shift-left: dbl[][] [] -> [w411]
              shift-right: [w408] -> w303
              shift-left: u32[] [] -> [w410]
              tunnel: w286 -> [w399]
              i -> [w401]
              stop <- w390 continue-if-true
              w406 = 1000.0 ("x")
              n287 = Increment(x=w422) -> (x+1=w421:i32)
              n288 = Equal To 0?(x=w401) -> (x = 0?=w400:bool)
              n289 = flat-sequence {
                tunnel: [w437] -> w420
                tunnel: w394 -> [w436]
                tunnel: [w435] -> w397
                tunnel: [w434] -> w418
                tunnel: w413 -> [w433]
                tunnel: [w432] -> w412
                frame #0 {
                  n290 = Tick Count (ms)() -> (millisecond timer value=w434:u32)
                  n291 = call "PSI9016 Read Stream Data.vi"("error in (no error)"=w433, "TCP connection ref in"=w436) -> ("sequence number"=w437:i32, "error out"=w432:errorcluster, "data"=w435:dbl[])  [unwired: 1 in, 2 out]
                }
              }
              n292 = Subtract(x=w418, y=w417) -> (x-y=w407:u32)
              n293 = case shown="True" w426 {
                tunnel: [w440 1] -> w425
                tunnel: w424 -> [w441 w442]
                tunnel: [w440 w442] -> w423
                frame False {
                  n294 = Decrement(x=w441) -> (x-1=w440:i32)
                }
                frame True {
                }
              }
              n295 = Multiply(x=w406, y=w416) -> (x*y=w415:dbl)
              n296 = Divide(x=w407, y=w406) -> (x/y=w398:dbl)
              n297 = Less?(x=w407, y=w415) -> (x < y?=w414:bool)
              n298 = local read "Runstop"() -> (w403:bool)
              n299 = case shown="True" w400 {
                tunnel: w399 -> [_ w431]
                tunnel: [w428 w430] -> w396
                tunnel: w398 -> [w428 w430]
                tunnel: [w427 w429] -> w395
                tunnel: w397 -> [w427 w429]
                frame False {
                }
                frame True {
                  n300 = Set Occurrence(w431) -> ()
                }
              }
              n301 = local read "EndVI"() -> (w393:bool)
              n302 = Build Array (concatenate)(w410, w398) -> (w408:dbl[])
              n303 = Build Array (concatenate)(w411, w397) -> (w409:dbl[][])
              n304 = Not Equal?(x=w420, y=w421) -> (x != y?=w419:bool)
              n305 = Not(x=w403) -> (.not. x?=w402:bool)
              n306 = Greater Than 0?(x=w425) -> (x > 0?=w405:bool)
              n307 = Not(x=w393) -> (.not. x?=w392:bool)
              n308 = case shown="True" w419 {
                frame False {
                }
                frame True {
                  n309 = local read "Missed Packets"() -> (w439:i8)
                  n310 = Increment(x=w439) -> (x+1=w438:i8)
                  n311 = local write "Missed Packets"(w438) -> ()
                }
              }
              n312 = And(x=w402, y=w405) -> (x .and. y?=w404:bool)
              n313 = And(x=w404, y=w414) -> (x .and. y?=w391:bool)
              n314 = local write "Samples Collected"(w420) -> ()
              n315 = local write "datumtime"(w396) -> ()
              n316 = local write "datumpressure"(w395) -> ()
              n317 = And(x=w391, y=w392) -> (x .and. y?=w390:bool)
            }
            n318 = local write "Running"(w302) -> ()
            n319 = local write "datatimes"(w303) -> ()
            n320 = local write "datapressure"(w281) -> ()
            n321 = call "PSI9016 Stop Stream.vi"("error in (no error)"=w295, "TCP connection ref in"=w290) -> ("error out"=w306:errorcluster)  [unwired: 3 in, 2 out]
            n322 = property on="unitselect" class="Ring (strict)"("Val(Sgnl)"=w304) -> ()  [unwired: 2 in, 2 out]
            n323 = property on="Run" class="Bool (strict)"("DisabledEnum"=w280, "Value"=w305) -> ()  [unwired: 2 in, 2 out]
            n324 = property on="Runstop" class="Bool (strict)"("Value"=w305, "DisabledEnum"=w307) -> ()  [unwired: 2 in, 2 out]
            n325 = property on="unlock" class="Bool (strict)"("Val(Sgnl)"=w308) -> ()  [unwired: 2 in, 2 out]
            n326 = call <vilib>:"Unset Busy.vi"("error in (no error)"=w306) -> ("error out"=w285:errorcluster)  [unwired: 10 in]
            n327 = property on="selectgraph2" class="Ring (strict)"("Val(Sgnl)"=w312) -> ()  [unwired: 2 in, 2 out]
            n328 = property on="Toggle 1-15" class="Bool (strict)"("DisabledEnum"=w280) -> ()  [unwired: 2 in, 2 out]
            n329 = property on="channelselect" class="Clust (strict)"("DisabledEnum"=w280) -> ()  [unwired: 2 in, 2 out]
            n330 = property on="Open save folder" class="Bool (strict)"("DisabledEnum"=w280) -> ()  [unwired: 2 in, 2 out]
            n331 = property on="selectgraph2" class="Ring (strict)"("DisabledEnum"=w280) -> ()  [unwired: 2 in, 2 out]
            n332 = property on="unitselect" class="Ring (strict)"("DisabledEnum"=w280) -> ()  [unwired: 2 in, 2 out]
            n333 = property on="EndVI" class="Bool (strict)"("DisabledEnum"=w280) -> ()  [unwired: 2 in, 2 out]
            n334 = property on="unlock" class="Bool (strict)"("DisabledEnum"=w280) -> ()  [unwired: 2 in, 2 out]
            n335 = property on="Rezero" class="Bool"("DisabledEnum"=w280) -> ()  [unwired: 2 in, 2 out]
            n336 = property on="Load past data:" class="Path"("DisabledEnum"=w280) -> ()  [unwired: 2 in, 2 out]
            n337 = property on="Folder path:" class="Path"("DisabledEnum"=w280) -> ()  [unwired: 2 in, 2 out]
          }
          frame #1 {
            n338 = local read "datumtime"() -> (w445:dbl)
            n339 = Greater?(x=w445, y=5.0) -> (0:w447:bool)
            n340 = Boolean To (0,1)(Boolean=w447) -> (0, 1=w444:i16)
            n341 = case shown="1" w444 {
              frame 0, Default {
              }
              frame 1 {
                n342 = local read "File prefix:"() -> (w460:string)
                n343 = local read "Folder path:"() -> (w456:path)
                n344 = local read "atmpressure"() -> (w451:dbl)
                n345 = local read "datapressure"() -> (w455:dbl[][])
                n346 = local read "datatimes"() -> (w454:dbl[])
                n347 = Concatenate Strings(w460, "_dummy") -> (w458:string)
                n348 = local read "run time"() -> (w457:timestamp)
                n349 = call "save_p_data.vi"("File prefix:"=w458, "run time"=w457, "Folder path:"=w456, "datapressure"=w455, "atmpressure"=w451, "datatimes"=w454) -> ("Saved file:"=w453:string, "Output folder:"=w449:path, "Folder \nchanged:"=w452:bool)  [unwired: 11 in]
                n350 = local write "Folder \nchange:"(w452) -> ()
                n351 = local write "Saved file:"(w453) -> ()
                n352 = local write "Folder path:"(w449) -> ()
                n353 = local write "Dummy \nsave:"(TRUE ("Dummy \nsave:")) -> ()
              }
            }
          }
        }
      }
      event "Open save folder": Value Change {
        n354 = event-data() -> ()  [unwired: 1 in, 6 out]
        n355 = local read "Folder path:"() -> (w463:path)
        n356 = call <vilib>:"Check if File or Folder Exists.vi"("path"=w463) -> ("file or folder exists?"=w461:bool, "dup path"=w462:path)  [unwired: 8 in, 1 out]
        n357 = case shown="False" w461 {
          tunnel: w462 -> [_ w465]
          frame False {
            n358 = call "Open save folder error message"() -> ()  [unwired: 10 in, 2 out]
          }
          frame True {
            n359 = call-poly <vilib>:"Open URL in Default Browser.vi"("path"=w465) -> ()  [unwired: 5 in, 2 out]
          }
        }
        n360 = property on="Open save folder" class="Bool (strict)"("Value"=FALSE) -> ()  [unwired: 2 in, 2 out]
      }
      event Timeout {
        n361 = event-data() -> ()  [unwired: 1 in, 2 out]
        n362 = local read "Connected"() -> (w468:bool)
        n363 = case shown="True" w468 {
          tunnel: [errorcluster {"status"=FALSE, "code"=0, "source"=""} ("error out") w479] -> w467
          frame False {
          }
          frame True {
            n364 = local read "TCPref"() -> (w478:refnum<k5>)
            n365 = call "PSI9016 Read Status.vi"("TCP connection ref in"=w478) -> ("error out"=w479:errorcluster)  [unwired: 4 in, 2 out]
          }
        }
        n366 = Unbundle By Name(w467) -> ("status"=w466:bool)
        n367 = case shown="True" w466 {
          frame False {
          }
          frame True {
            w470 = T2."Disabled and Grayed Out" ("Disabled")
            n368 = local write "Connected"(FALSE ("Connected")) -> ()
            n369 = One Button Dialog(message="Connection Failed!") -> ()  [unwired: 1 in, 1 out]
            n370 = property on="Run" class="Bool (strict)"("DisabledEnum"=w470) -> ()  [unwired: 2 in, 2 out]
            n371 = property on="Rezero" class="Bool"("DisabledEnum"=w470) -> ()  [unwired: 2 in, 2 out]
            n372 = property on="Connect" class="Bool (strict)"("BoolText.Text"="Connect" ("Boolean Text.Text"), "BoolText.TextColor"=u32 0, "Value"=FALSE ("Connect"), "DisabledEnum"=T2."Enabled" ("Disabled")) -> ()  [unwired: 2 in, 2 out]
          }
        }
      }
    }
    n373 = call <vilib>:"General Error Handler.vi"("type of dialog (OK msg:1)"=3, "error in (no error)"=w19) -> ("error?"=w14:bool)  [unwired: 9 in, 4 out]
    n374 = case shown="True" w14 {
      selector: w14 -> [_ w20]
      frame False {
      }
      frame True {
        n375 = property on="EndVI" class="Bool (strict)"("Val(Sgnl)"=w20) -> ()  [unwired: 2 in, 2 out]
      }
    }
  }
  "Missed Packets" <- i8 0 ("Missed Packets")
  "Dummy \nsave:" <- w3
  "Folder \nchange:" <- w3
  "Load feedback" <- w1
